vi "GOOP_ClassTool.vi"(0 "ClassRef":refnum<vi>, 5 "Error In":errorcluster) -> (19 "Error Out":errorcluster)   [LabVIEW 2020]
uses:
  ClassProviders/Common/ScriptingFunctions/Scripting_ConnectorPanePatternType.ctl
  <vilib>/Utility/miscctls.llb/LVPositionTypeDef.ctl
  API/GDSAPI_CreateInterfaceType.ctl
  ClassProviders/Provider_BaseClassInterface/ClassWriter_class/InterfaceMethodsToCreate.ctl
  ClassProviders/Common/CommonVIs/CommonVIs_AttributeType.ctl
  ClassProviders/Common/CommonVIs/CommonVIs_AttributeDataType.ctl
  ClassProviders/Common/String/GDSString_AccessScopeModifierType.ctl
  ClassProviders/Provider_EndevoGOOP300/GOOP300_SubVIs/GOOP300_MethodScopeType.ctl
  API/GDSAPI_SubVIs/GDSAPI_MethodType.ctl
  <vilib>/regexp/Match Regular Expression.xnode
  ClassProviders/Common/ScriptingFunctions/Scripting.lvclass
  ClassProviders/Provider_BaseClassInterface/ClassWriter_class/ClassWriter.lvclass
panel:
  in  "SelectAll":bool
  in  "ClassesCancel":bool
  in  "ClassesOK":bool
  in  "Classes":i32[](listbox)
  in  "MoreClasses":bool
  in  "Class(es)":u16(ring) items=["<Select Class(s)>", "-"]
  in  "Tab":enum32{"CP", "ClassControlName", "Interface"}(tab)
  in  "ApplyCP":bool
  in  "CP2":u16(ring) caption="To" items=["4x4x4", "5x6x5", "6x8x6"]
  out "CP1":T1 caption="From" items=["4x4x4", "5x6x5", "6x8x6"]
  out "ClassNameOut":string
  out "ClassNameIn":string
  in  "ClassControlName":string(combo) caption="New names of class controls and indicators"
  in  "UpdateClassControlNames":bool
  in  "InterfaceToCreate":u16(ring) caption="Select interface to create from current class..." items=["Create a parent class based on some of my methods of my class: AA", "Create an Interface(By VI Server) based on some of my methods of my class: AA", "Create an Interface and Adaptor class based on some of my methods of my class: AA"]
  out "InterfaceOptionTab":enum32{"Parent", "Adapter"}(tab)
  out "ReasonWhyParentClassCan'tBeCreated":string
  in  "CreateClassAndMethods":bool
  in  "ParentFolder":path
  in  "ParentClassName":string
  in  "ParentClass":u16(ring) items=["", "A", "AA-Base", "ABC", "B", "Base", "ClassWriter", "ClassWriterGOOP300", "ClassWriterGOOP400", "ClassWriterNative", "Scripting"]
  out "MyClassName(ParentClass)":string
  in  "MyClassMethods":i32[](listbox) caption="Class methods to add in the Parent class"
  out "Parent/InterafaceImage":u16(ring)
  in  "ParentMethodName":string
  out "MyClassName(InteraceClass)":string
  in  "AdaptorClassName":string
  in  "AdaptorFolder":path
  in  "Parent Methods":i32(listbox)
  in  "MyClassMethods(Interface)":i32[](listbox) caption="Class methods"
  in  "InterfaceClassName":string
  in  "InterfaceClass":u16(ring) items=["", "A", "B", "BBB", "CCC", "ClassWriter", "ClassWriterGOOP300", "ClassWriterGOOP400", "ClassWriterNative", "IA", "Scripting", "Top"]
  in  "InterfaceFolder":path
  out "ReasonWhyInterfaceClassCan'tBeCreated":string
  in  "CreateInterfaceAdaptorClassAndMethods":bool
  # "Select the Connector Pane you wish to change to and press CHANGE when done."
  # "Change the class reference control and indicator name. Press UPDATE when done."
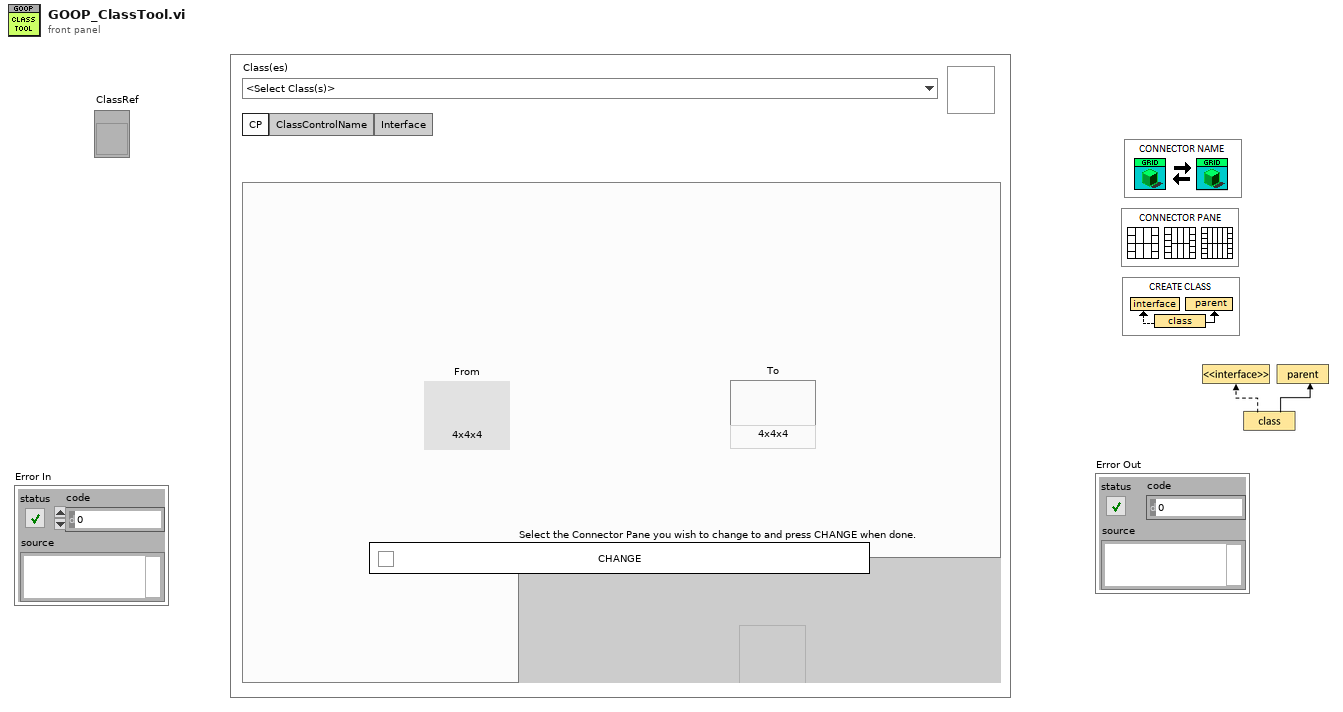
[diagram p1: front panel]
types:
  T1 = typedef "Scripting_ConnectorPanePatternType.ctl" = u16
  T2 = cluster{"Classes":refnum<vi>[], "Selected":i32[], "DropDownClasses":refnum<vi>[], "Interfaces":refnum<vi>[], "Methods":refnum<vi>[], "ExistingParentClassIdx":i32, "NewDropDownClassIdx":i32, "AdpUpdates":bool, "SelectClassPath":path, "ParentClassCreated":path, "NewClassCreated":bool}
  T3 = enum32{"Invalid", "Default", "Floating", "Floating/Auto-Hide", "Modal"}
  T4 = enum8{"Enabled", "Disabled", "Disabled and Grayed Out"}
  T5 = enum32{"invalid scope", "public", "private", "protected", "community"}
  T6 = typedef "LVPositionTypeDef.ctl" = cluster{"Left":i32, "Top":i32}
  T7 = typedef "GDSAPI_CreateInterfaceType.ctl" = cluster{"NewInterfaceFolder":path, "InterfaceName":string, "InterfaceDescription":string, "ParentInterfacesFilePath":path[], "FolderSuffix":string, "MethodsToCreate":T8[]}
  T8 = typedef "ClassWriter.lvclass/InterfaceMethodsToCreate.ctl" = cluster{"Name":string, "Description":string, "MethodsArgumentsIn":T9[], "MethodsArgumentsOut":T9[], "DecendantsMustOverride":bool}
  T9 = typedef "CommonVIs_AttributeType.ctl" = cluster{"Name":string, "DataType":T10, "ArrayDim":i32, "CtrlPath":path, "DataTypeString":string, "AccessScope":T11, "InitialData":variant}
  T10 = typedef "CommonVIs_AttributeDataType.ctl" = enum16{"UINT8", "INT8", "UINT16", "INT16", "UINT32", "INT32", "UINT64", "INT64", "SGL", "DBL", "EXT", "CSG", "CDB", "CXT", "TimeStamp", "STRING", "PATH", "BOOL", "ENUM", "RefNum", "VIRefNum", "LabVIEW Class", "Cluster", "Variant", "TypeDef", "Waveform", "LabVIEW Object", "Other", "void", "Set", "Map"}
  T11 = typedef "GDSString_AccessScopeModifierType.ctl" = enum16{"public", "private", "protected", "internal"}
  T12 = typedef "GOOP300_MethodScopeType.ctl" = enum16{"Use Parent Folder Scope", "Public", "Protected", "Private", "Community"}
  T13 = typedef "GDSAPI_MethodType.ctl" = enum16{"Read Attribute", "Write Attribute", "Read & Write Attribute", "None Modifying Method", "Get Property", "Set Property", "Read Property", "Write Property", "Static Method", "Interface Method"}
  T14 = cluster{"MethodName":string, "RelativeMethodPath":path, "MethodDescription":string, "Scope/Visibility":T12, "MethodType":T13, "RelativeProjectClassPath":string, "DynamicDispatchVi":bool, "OverrideMethod(Path)/PropertyMethod(AttributeName)":string}
  T15 = typedef "GDSLvCLass_ClassSettingsType.ctl" = cluster{"ClassProviderName":string, "ClassTemplateUsed":string, "ClassTemplateVersion":string, "ClassDescription":string, "PlugIns":T16[], "ConnectorPanePattern":string}
  T16 = typedef "GDSLvClass_PlugIn.ctl" = cluster{"Type":T17, "ID":string, "Version":string, "Path":path, "Name":string, "Data":variant}
  T17 = typedef "GDSLvClass_PlugInTypes.ctl" = enum16{"DesignPattern", "MethodTypes"}
  T18 = cluster{"result string":string, "ClassRef":refnum<vi>}
  T19 = cluster{"result string":string, "ClassRef":refnum<vi>}[]
  T20 = typedef "lveventtype.ctl" = enum32{"Null", "Timeout", "Annotation Menu Selection", "Annotation Menu Selection?", "App Instance Close", "App Instance Close?", "Autoscale Range Change", "Bookmark Info Change", "Cell Edit", "Cell Edit?", "Cursor Grab", "Cursor Grab?", "Cursor Menu Selection", "Cursor Menu Selection?", "Cursor Move", "Cursor Release", "Data Change", "Direction Change", "Display State Change", "Drag Ended", "Drag Enter", "Drag Leave", "Drag Over", "Drag Source Update", "Drag Starting", "Drag Starting?", "Drop", "Exec State Change", "Key Down", "Key Down?", "Key Repeat", "Key Repeat?", "Key Up", "Listbox Double Click", "Menu Activation?", "Menu Selection (App)", "Menu Selection? (App)", "Menu Selection (User)", "Mouse Down", "Mouse Down?", "Mouse Enter", "Mouse Leave", "Mouse Move", "Mouse Up", "Mouse Wheel", "NI Security User Change (App)", "Pane Size", "Panel Close", "Panel Close?", "Panel Resize", "Plot Attribute Change", "Scale Range Change", "Shortcut Menu Activation?", "Shortcut Menu Selection (App)", "Shortcut Menu Selection? (App)", "Shortcut Menu Selection (User)", "Tree Double Click", "Tree Drag", "Tree Drag?", "Tree Drop", "Tree Drop?", "Tree Item Close", "Tree Item Close?", "Tree Item Open", "Tree Item Open?", "User Event", "Value Change"}
  T21 = typedef "LVRowAndColumnUnsignedTypeDef.ctl" = cluster{"Row":u32, "Column":u32}
  T22 = cluster{"MethodName":string, "RelativeMethodPath":path, "MethodDescription":string, "Scope/Visibility":T12, "MethodType":T13, "RelativeProjectClassPath":string, "DynamicDispatchVi":bool, "OverrideMethod(Path)/PropertyMethod(AttributeName)":string}[]
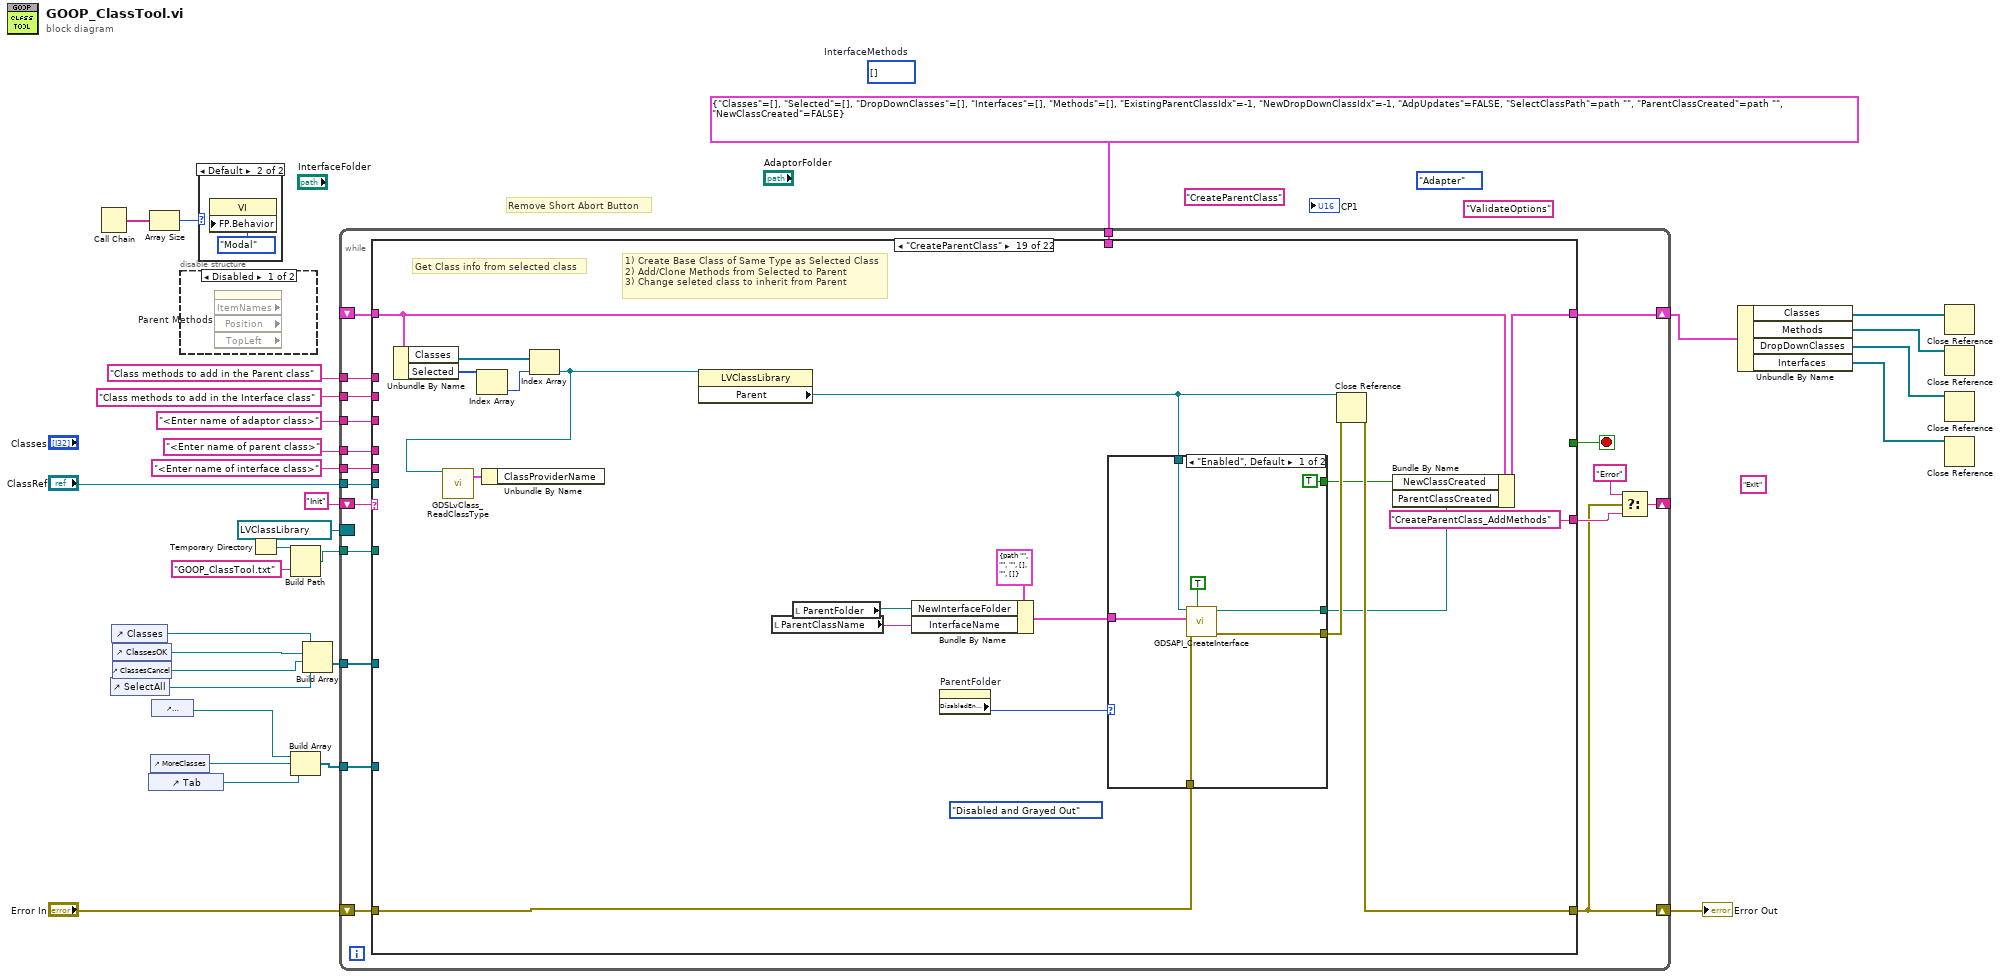
[diagram p0: block diagram]
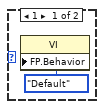
[diagram p3: hidden frame]
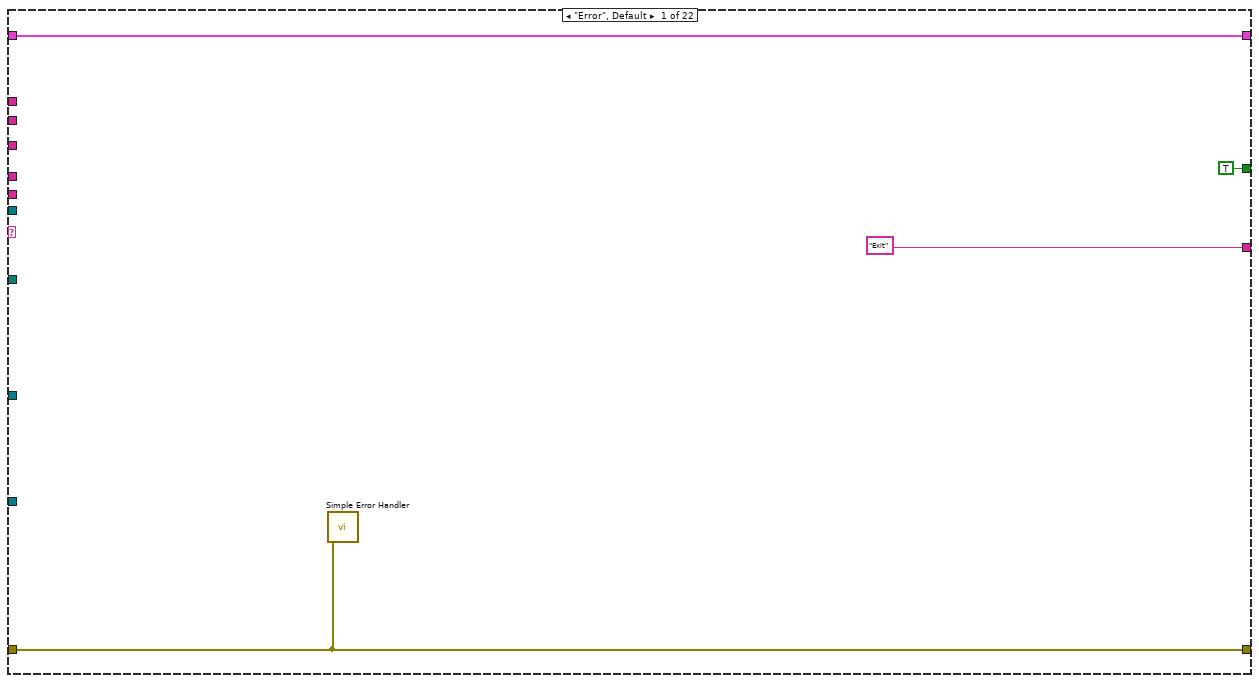
[diagram p4: hidden frame]
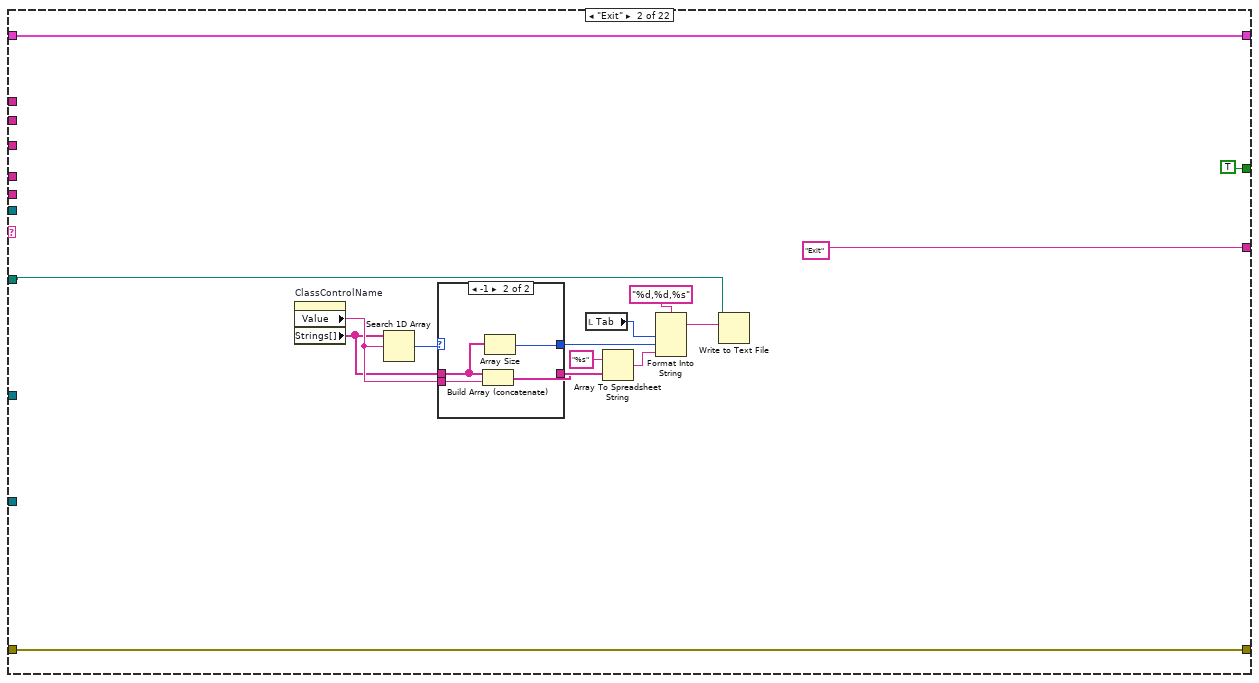
[diagram p5: hidden frame]
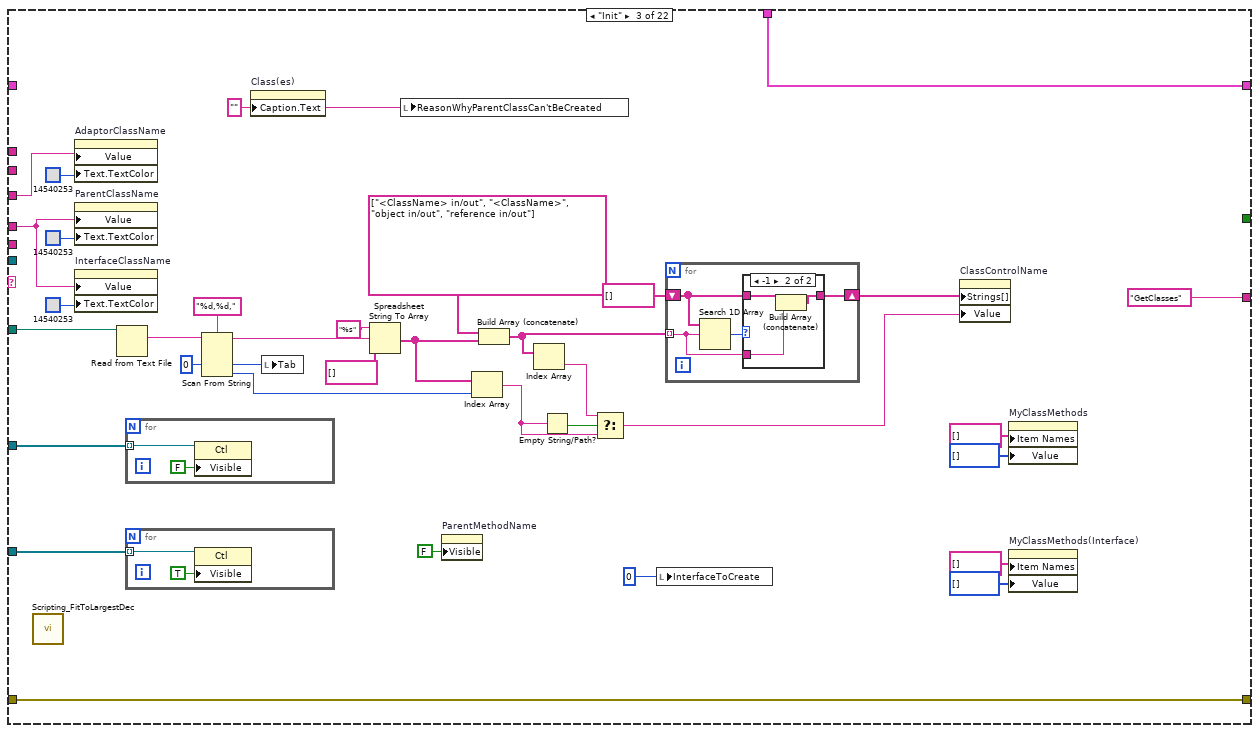
[diagram p7: hidden frame]
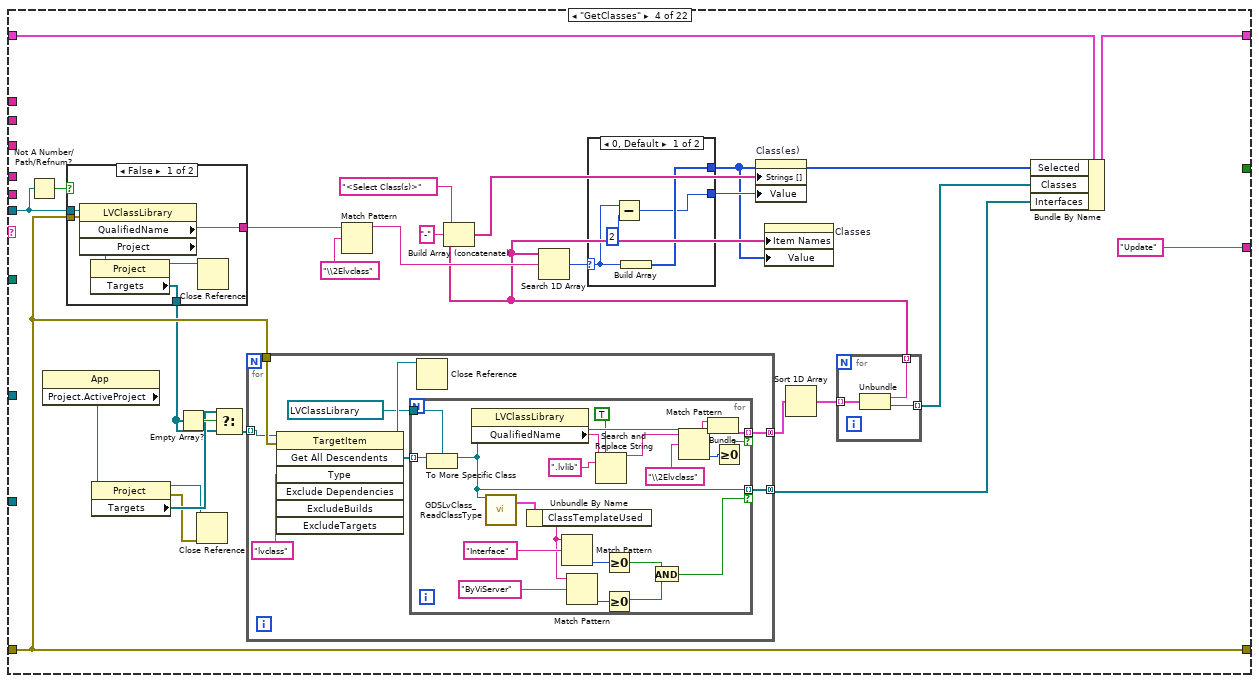
[diagram p9: hidden frame]
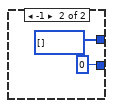
[diagram p10: hidden frame]
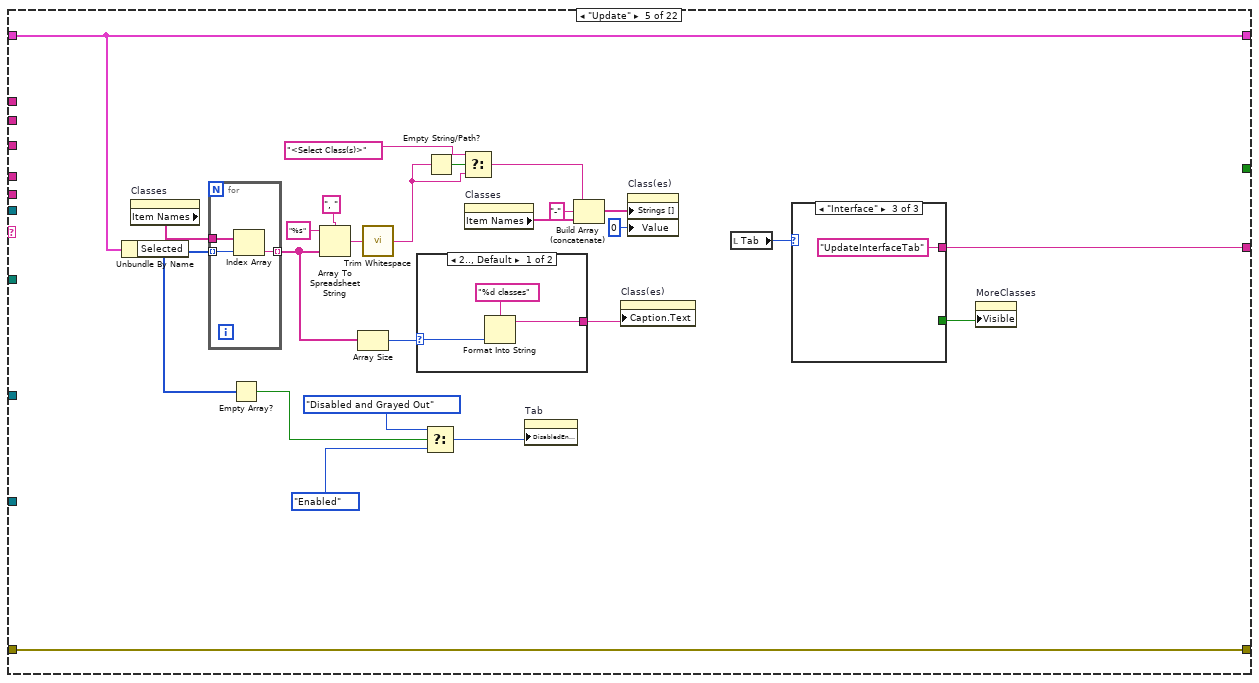
[diagram p12: hidden frame]
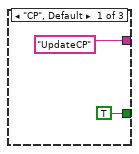
[diagram p13: hidden frame]
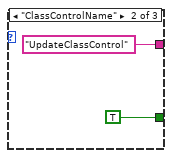
[diagram p14: hidden frame]
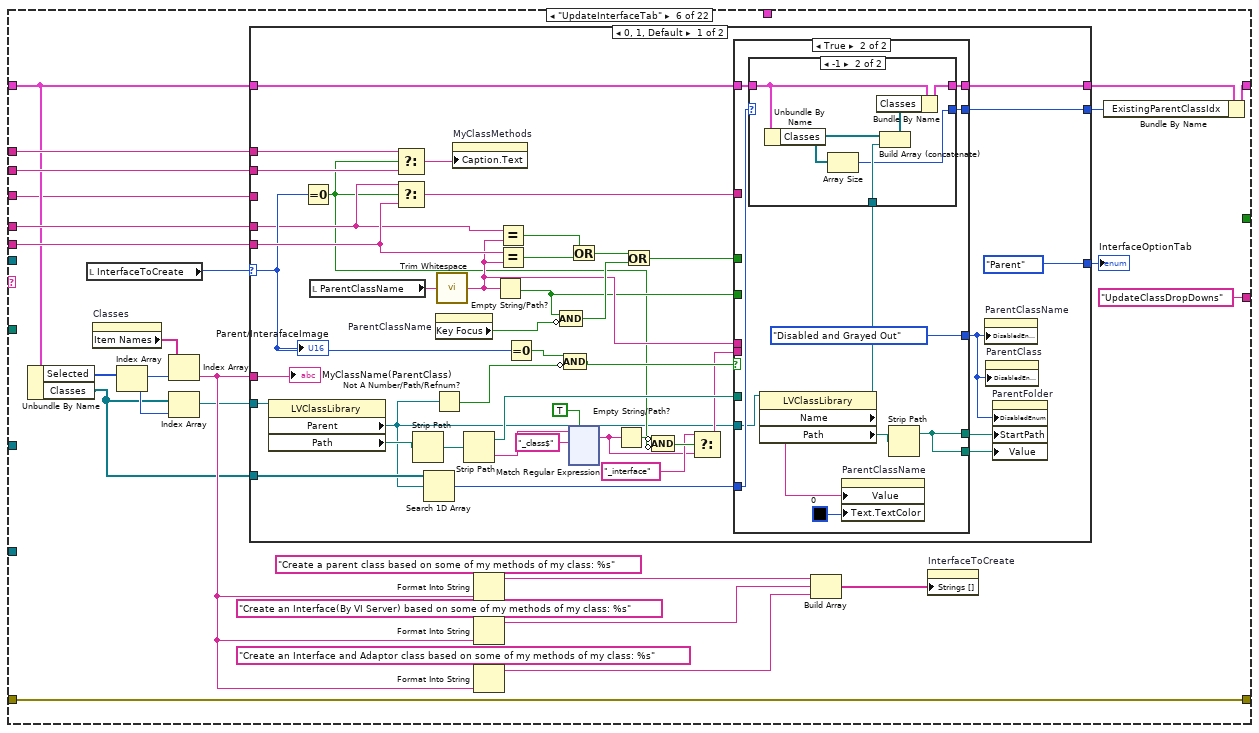
[diagram p16: hidden frame]
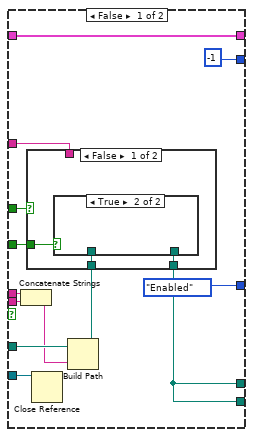
[diagram p17: hidden frame]
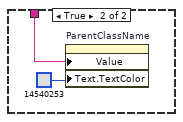
[diagram p19: hidden frame]
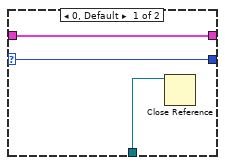
[diagram p20: hidden frame]
diagram:
  (unwired) "Exit"
  (unwired) "CreateParentClass"
  (unwired) "ValidateOptions"
  (unwired) enum32{"Parent", "Adapter"}."Adapter" ("InterfaceOptionTab")
  (unwired) i32[] []  # InterfaceMethods
  # "Remove Short Abort Button"
  n1 = Call Chain() -> (call chain=w7:string[])
  n2 = control-ref of="SelectAll"() -> (w18:refnum<vi>)
  n3 = control-ref of="Classes"() -> (w27:refnum<vi>)
  n4 = control-ref of="ClassesOK"() -> (w26:refnum<vi>)
  n5 = control-ref of="ClassesCancel"() -> (w25:refnum<vi>)
  n6 = control-ref of="Tab"() -> (w22:refnum<vi>)
  n7 = Array Size(array=w7) -> (size(s)=w6:i32)
  n8 = control-ref of="MoreClasses"() -> (w23:refnum<vi>)
  n9 = control-ref of="Class(es)"() -> (w17:refnum<vi>)
  n10 = disable-structure shown="Disabled" {
    frame Disabled {
      n11 = property on="Parent Methods" class="MCListbox (strict)" props=["ItemNames", "Position", "TopLeft"]() -> ()  [unwired: 2 in, 5 out]
    }
    frame Enabled {
    }
  }
  n12 = case shown="Default" w6 {
    frame 1 {
      n13 = property class="VI"("FP.Behavior"=T3."Default" ("Front Panel Window:Behavior")) -> ()  [unwired: 2 in, 2 out]
    }
    frame Default {
      n14 = property class="VI"("FP.Behavior"=T3."Modal" ("Front Panel Window:Behavior")) -> ()  [unwired: 2 in, 2 out]
    }
  }
  n15 = Temporary Directory() -> (w14:path)
  n16 = Build Path(base path=w14, name or relative path="GOOP_ClassTool.txt") -> (appended path=w13:path)
  n17 = Build Array(w17, w23, w22) -> (w21:refnum<vi>[])
  n18 = Build Array(w27, w26, w25, w18) -> (w24:refnum<vi>[])
  n19 = while {
    shift-right: [w46] -> w28
    shift-left: "Error In" -> [w51]
    shift-right: [w49] -> _
    shift-left: "Init" -> [w50]
    shift-right: [w45] -> w1
    shift-left: _ -> [w44]
    tunnel: w24 -> [w43]
    tunnel: w21 -> [w42]
    tunnel: "ClassRef" -> [w41]
    tunnel: T2 {"Classes"=[], "Selected"=[], "DropDownClasses"=[], "Interfaces"=[], "Methods"=[], "ExistingParentClassIdx"=-1, "NewDropDownClassIdx"=-1, "AdpUpdates"=FALSE, "SelectClassPath"=path "", "ParentClassCreated"=path "", "NewClassCreated"=FALSE} -> [w40]
    tunnel: w13 -> [w39]
    tunnel: "<Enter name of parent class>" ("ParentClassName") -> [w37]
    tunnel: "<Enter name of interface class>" ("ParentClassName") -> [w36]
    tunnel: "Class methods to add in the Parent class" ("Caption.Text") -> [w35]
    tunnel: "Class methods to add in the Interface class" ("Caption.Text") -> [w34]
    border: refnum<vi> refnum ("ClassRef") -> [_]
    tunnel: "<Enter name of adaptor class>" ("ParentClassName") -> [w33]
    stop <- w38 stop-if-true
    n20 = case shown="\"CreateParentClass\"" w50 {
      tunnel: w51 -> [w52 w70 w110 w133 w220 w247 w641 w722 w772 w799 w939 w1053 w1102 w1477 w1486 w1504 w1546 w1671 w1678 w1712 w1740 w1749]
      tunnel: [w52 w70 w110 w133 w220 w247 w641 w722 w772 w799 w939 w1053 w1102 w1477 w1483 w1500 w1546 w1671 w1685 w1706 w1733 w1749] -> w46
      tunnel: ["Exit" "Exit" "GetClasses" "Update" w208 "UpdateClassDropDowns" "UpdateMethods" w710 "AutoUpdateAdaptorName" "ValidateOptions" _ _ w1103 "Update" "Done" "Done" _ _ "CreateParentClass_AddMethods" w1709 "Done" ("message") "Exit"] -> w47
      tunnel: [w54 w68 w107 w136 w209 w236 w640 w718 w773 w798 w937 w1052 w1104 w1478 w1487 w1507 w1545 w1672 w1684 w1708 w1731 w1747] -> w45
      tunnel: w44 -> [w54 w68 _ w149 w209 w235 w638 w719 w773 w798 w937 w1052 w1099 w1480 w1487 w1507 w1545 w1672 w1690 w1708 w1731 w1747]
      tunnel: w43 -> [_ _ w109 _ _ _ _ _ _ _ _ _ w1101 _ _ _ _ _ _ _ _ _]
      tunnel: w42 -> [_ _ w108 _ _ _ _ _ _ _ _ _ w1100 _ _ _ _ _ _ _ _ _]
      tunnel: w41 -> [_ _ _ w132 _ _ _ _ _ _ _ _ _ _ _ _ _ _ _ _ _ _]
      tunnel: w40 -> [_ _ w107 _ _ _ _ _ _ _ _ _ _ _ _ _ _ _ _ _ _ _]
      tunnel: w39 -> [_ w57 w99 _ _ _ _ _ _ _ _ _ _ _ _ _ _ _ _ _ _ _]
      tunnel: [TRUE TRUE _ _ _ _ _ _ _ _ _ _ _ _ _ _ _ _ _ _ _ _] -> w38
      tunnel: w37 -> [_ _ w81 _ _ w246 _ _ _ w796 w936 _ w1098 _ _ _ _ _ _ _ _ _]
      tunnel: w36 -> [_ _ _ _ _ w243 _ _ _ _ w935 _ w1096 _ _ _ _ _ _ _ _ _]
      tunnel: w35 -> [_ _ _ _ _ w239 _ _ _ _ _ _ _ _ _ _ _ _ _ _ _ _]
      tunnel: w34 -> [_ _ _ _ _ w238 _ _ _ _ _ _ _ _ _ _ _ _ _ _ _ _]
      tunnel: w33 -> [_ _ w78 _ _ w232 _ _ _ w795 _ _ w1095 _ _ _ _ _ _ _ _ _]
      frame "Error", Default {
        n21 = call <vilib>:"Simple Error Handler.vi"("error in (no error)"=w52) -> ()  [unwired: 4 in, 5 out]
      }
      frame "Exit" {
        n22 = property on="ClassControlName" class="CmbBox"() -> ("Value"=w62:string, "Strings[]"=w61:string[])  [unwired: 2 in, 2 out]
        n23 = Search 1D Array(1D array=w61, element=w62) -> (index of element=w58:i32)  [unwired: 1 in]
        n24 = case shown="-1" w58 {
          selector: w58 -> [w72 _]
          tunnel: [w72 w74] -> w59
          tunnel: w61 -> [w71 w75]
          tunnel: w62 -> [_ w76]
          tunnel: [w71 w73] -> w65
          frame 0, Default {
          }
          frame -1 {
            n25 = Build Array (concatenate)(w75, w76) -> (w73:string[])
            n26 = Array Size(array=w75) -> (size(s)=w74:i32)
          }
        }
        n27 = local read "Tab"() -> (w67:enum32{"CP", "ClassControlName", "Interface"})
        n28 = Array To Spreadsheet String(array=w65, 3:"%s" ("format string")) -> (spreadsheet string=w64:string)  [unwired: 1 in]
        n29 = Format Into String(format string="%d,%d,%s", w67, w59, w64) -> (resulting string=w66:string)  [unwired: 2 in, 1 out]
        n30 = Write to Text File(file (use dialog)=w57, text=w66) -> ()  [unwired: 2 in, 3 out]
      }
      frame "Init" {
        w80 = "" ("Caption.Text")
        n31 = call "Scripting_FitToLargestDec.vi"() -> ()  [unwired: 6 in, 2 out]
        n32 = property on="AdaptorClassName" class="Str"("Value"=w78, "Text.TextColor"=u32 14540253) -> ()  [unwired: 2 in, 2 out]
        n33 = property on="ParentClassName" class="Str"("Value"=w81, "Text.TextColor"=u32 14540253) -> ()  [unwired: 2 in, 2 out]
        n34 = property on="InterfaceClassName" class="Str"("Value"=w81, "Text.TextColor"=u32 14540253) -> ()  [unwired: 2 in, 2 out]
        n35 = Read from Text File(file (use dialog)=w99) -> (text=w106:string)  [unwired: 3 in, 3 out]
        n36 = for {
          tunnel: w109 -> [w123] mode=indexing
          n37 = property on="Property Node" class="Ctl"(reference=w123, "Visible"=FALSE) -> ()  [unwired: 1 in, 2 out]
        }
        n38 = for {
          tunnel: w108 -> [w121] mode=indexing
          n39 = property on="Property Node" class="Ctl"(reference=w121, "Visible"=TRUE) -> ()  [unwired: 1 in, 2 out]
        }
        n40 = Scan From String(format string="%d,%d,", input string=w106, default 1=0 ("default value 1")) -> (remaining string=w104:string, output 1=w97:i32, output 2=w95:i32)  [unwired: 3 in, 2 out]
        n41 = property on="Class(es)" class="Ring (strict)"("Caption.Text"=w80) -> ()  [unwired: 2 in, 2 out]
        n42 = local write "Tab"(w97) -> ()
        n43 = Spreadsheet String To Array(format string="%s", spreadsheet string=w104, array type (2D Dbl)=string[] []) -> (array=w96:string[])  [unwired: 1 in]
        n44 = local write "ReasonWhyParentClassCan'tBeCreated"(w80) -> ()
        n45 = property on="ParentMethodName" class="Str"("Visible"=FALSE) -> ()  [unwired: 2 in, 2 out]
        n46 = Index Array(array=w96, index=w95) -> (element=w90:string)
        n47 = Build Array (concatenate)(string[] ["<ClassName> in/out", "<ClassName>", "object in/out", "reference in/out"] ("Strings []"), w96) -> (w93:string[])
        n48 = Index Array(array=w93) -> (element=w91:string)  [unwired: 1 in]
        n49 = Empty String/Path?(string/path=w90) -> (empty?=w92:bool)
        n50 = Select(t=w91, s=w92, f=w90) -> (s? t:f=w89:string)
        n51 = local write "InterfaceToCreate"(0) -> ()
        n52 = for {
          tunnel: w93 -> [w113] mode=indexing
          shift-right: [w112] -> w94
          shift-left: string[] [] -> [w114]
          n53 = Search 1D Array(1D array=w114, element=w113) -> (index of element=w115:i32)  [unwired: 1 in]
          n54 = case shown="-1" w115 {
            tunnel: w114 -> [w116 w119]
            tunnel: w113 -> [_ w118]
            tunnel: [w116 w117] -> w112
            frame 0, Default {
            }
            frame -1 {
              n55 = Build Array (concatenate)(w119, w118) -> (w117:string[])
            }
          }
        }
        n56 = property on="ClassControlName" class="CmbBox"("Strings[]"=w94, "Value"=w89) -> ()  [unwired: 2 in, 2 out]
        n57 = property on="MyClassMethods" class="LstBox (strict)"("Item Names"=string[] [], "Value"=i32[] [] ("MyClassMethods")) -> ()  [unwired: 2 in, 2 out]
        n58 = property on="MyClassMethods(Interface)" class="LstBox (strict)"("Item Names"=string[] [], "Value"=i32[] [] ("MyClassMethods")) -> ()  [unwired: 2 in, 2 out]
      }
      frame "GetClasses" {
        n59 = Not A Number/Path/Refnum?(number/path/refnum=w132) -> (NaN/Path/Refnum?=w131:bool)
        n60 = property class="App"() -> ("Project.ActiveProject"=w130:refnum<vi>)  [unwired: 2 in, 2 out]
        n61 = case shown="False" w131 {
          tunnel: [w162 _] -> w148
          tunnel: [w160 _] -> w129
          tunnel: w133 -> [w159 _]
          tunnel: w132 -> [w158 _]
          frame False {
            n62 = property class="LVClassLibrary"(reference=w158, error in=w159) -> ("QualifiedName"=w162:string, "Project"=w161:refnum<vi>)  [unwired: 2 out]
            n63 = property class="Project"(reference=w161) -> (reference out=w157:refnum<vi>, "Targets"=w160:refnum<vi>[])  [unwired: 1 in, 1 out]
            n64 = Close Reference(reference=w157) -> ()  [unwired: 1 in, 1 out]
          }
          frame True {
          }
        }
        n65 = property class="Project"(reference=w130) -> (reference out=w125:refnum<vi>, error out=w126:errorcluster, "Targets"=w141:refnum<vi>[])  [unwired: 1 in]
        n66 = Empty Array?(array=w129) -> (empty?=w142:bool)
        n67 = Close Reference(reference=w125, error in (no error)=w126) -> ()  [unwired: 1 out]
        n68 = Select(t=w141, s=w142, f=w129) -> (s? t:f=w140:refnum<vi>[])
        n69 = for {
          tunnel: [w171] -> w144 mode=concatenating
          tunnel: w133 -> [w170]
          tunnel: w140 -> [w169] mode=indexing
          tunnel: [w166] -> w124 mode=concatenating
          n70 = invoke class="TargetItem" method="Get All Descendents"(reference=w169, error in=w170, "Type"="lvclass") -> (reference out=w168:refnum<vi>, "All Descendents"=w172:refnum<vi>[])  [unwired: 4 in, 5 out]
          n71 = for {
            tunnel: w172 -> [w195] mode=indexing
            tunnel: [w189] -> w171 mode=indexing if=w192
            tunnel: refnum<vi> refnum ("ClassRef") -> [w184]
            tunnel: [w175] -> w166 mode=indexing if=w174
            n72 = To More Specific Class(target class=w184, reference=w195) -> (specific class reference=w175:refnum<vi>)  [unwired: 1 in, 1 out]
            n73 = property class="LVClassLibrary"(reference=w175) -> (reference out=w190:refnum<vi>, "QualifiedName"=w188:string)  [unwired: 1 in, 1 out]
            n74 = call "GDSLvClass_ReadClassType.vi"("Class Refnum In"=w175) -> ("ClassSettings"=w181:T15)  [unwired: 16 in, 2 out]
            n75 = Unbundle By Name(w181) -> ("ClassTemplateUsed"=w178:string)
            n76 = Match Pattern(string=w178, regular expression="Interface") -> (offset past match=w179:i32)  [unwired: 1 in, 3 out]
            n77 = Match Pattern(string=w178, regular expression="ByViServer") -> (offset past match=w176:i32)  [unwired: 1 in, 3 out]
            n78 = Search and Replace String(replace all?=TRUE ("replace all? (F)"), input string=w188, search string=".lvlib" ("regular expression")) -> (result string=w187:string)  [unwired: 5 in, 3 out]
            n79 = Greater Or Equal To 0?(x=w179) -> (x >= 0?=w182:bool)
            n80 = Greater Or Equal To 0?(x=w176) -> (x >= 0?=w183:bool)
            n81 = And(x=w182, y=w183) -> (x .and. y?=w174:bool)
            n82 = Match Pattern(string=w187, regular expression="\\2Elvclass") -> (before substring=w191:string, offset past match=w193:i32)  [unwired: 1 in, 2 out]
            n83 = Bundle("result string"=w191, "ClassRef"=w190) -> (w189:T18)  [unwired: 1 in]
            n84 = Greater Or Equal To 0?(x=w193) -> (x >= 0?=w192:bool)
          }
          n85 = Close Reference(reference=w168) -> ()  [unwired: 1 in, 1 out]
        }
        n86 = Match Pattern(string=w148, regular expression="\\2Elvclass") -> (before substring=w139:string)  [unwired: 1 in, 3 out]
        n87 = Sort 1D Array(array=w144) -> (sorted array=w138:T19)
        n88 = for {
          tunnel: w138 -> [w165] mode=indexing
          tunnel: [w164] -> w135 mode=indexing
          tunnel: [w163] -> w137 mode=indexing
          n89 = Unbundle(w165) -> ("result string"=w163:string, "ClassRef"=w164:refnum<vi>)
        }
        n90 = Build Array (concatenate)("<Select Class(s)>" ("element"), "-" ("element"), w137) -> (w145:string[])
        n91 = Search 1D Array(1D array=w137, element=w139) -> (index of element=w128:i32)  [unwired: 1 in]
        n92 = case shown="0, Default" w128 {
          selector: w128 -> [w154 _]
          tunnel: [w151 0 ("Classes")] -> w143
          tunnel: [w153 i32[] [] ("Classes")] -> w127
          frame 0, Default {
            n93 = Subtract(x=w154, y=2) -> (x-y=w151:i32)
            n94 = Build Array(w154) -> (w153:i32[])
          }
          frame -1 {
          }
        }
        n95 = property on="Class(es)" class="Ring (strict)"("Strings []"=w145, "Value"=w143) -> ()  [unwired: 2 in, 2 out]
        n96 = property on="Classes" class="LstBox (strict)"("Item Names"=w137, "Value"=w127) -> ()  [unwired: 2 in, 2 out]
        n97 = Bundle By Name(cluster=w149, "Selected"=w127, "Classes"=w135, "Interfaces"=w124) -> (w136:T2)
      }
      frame "Update" {
        n98 = Unbundle By Name(w209) -> ("Selected"=w207:i32[])
        n99 = property on="Classes" class="LstBox (strict)"() -> ("Item Names"=w219:string[])  [unwired: 2 in, 2 out]
        n100 = for {
          tunnel: w207 -> [w231] mode=indexing
          tunnel: w219 -> [w230]
          tunnel: [w229] -> w196 mode=indexing
          n101 = Index Array(array=w230, index=w231) -> (element=w229:string)
        }
        n102 = Empty Array?(array=w207) -> (empty?=w206:bool)
        n103 = Array To Spreadsheet String(delimiter (Tab)=", ", array=w196, 3:"%s" ("format string")) -> (spreadsheet string=w216:string)
        n104 = Array Size(array=w196) -> (size(s)=w215:i32)
        n105 = call <vilib>:"Trim Whitespace.vi"("string"=w216) -> ("trimmed string"=w200:string)  [unwired: 1 in]
        n106 = case shown="2.., Default" w215 {
          selector: w215 -> [w228 _]
          tunnel: [w226 _] -> w214
          frame 2.., Default {
            n107 = Format Into String(format string="%d classes", w228) -> (resulting string=w226:string)  [unwired: 2 in, 1 out]
          }
          frame ..1 {
          }
        }
        n108 = Select(t=T4."Disabled and Grayed Out", s=w206, f=T4."Enabled" ("Disabled")) -> (s? t:f=w203:T4)
        n109 = Empty String/Path?(string/path=w200) -> (empty?=w202:bool)
        n110 = Select(t="<Select Class(s)>" ("element"), s=w202, f=w200) -> (s? t:f=w199:string)
        n111 = property on="Classes" class="LstBox (strict)"() -> ("Item Names"=w213:string[])  [unwired: 2 in, 2 out]
        n112 = property on="Tab" class="TabCtl (strict)"("DisabledEnum"=w203) -> ()  [unwired: 2 in, 2 out]
        n113 = Build Array (concatenate)(w199, "-" ("element"), w213) -> (w212:string[])
        n114 = property on="Class(es)" class="Ring (strict)"("Caption.Text"=w214) -> ()  [unwired: 2 in, 2 out]
        n115 = property on="Class(es)" class="Ring (strict)"("Strings []"=w212, "Value"=0 ("Classes")) -> ()  [unwired: 2 in, 2 out]
        n116 = local read "Tab"() -> (w198:enum32{"CP", "ClassControlName", "Interface"})
        n117 = case shown="\"Interface\"" w198 {
          tunnel: ["UpdateCP" "UpdateClassControl" "UpdateInterfaceTab"] -> w208
          tunnel: [TRUE TRUE _] -> w197
          frame "CP", Default {
          }
          frame "ClassControlName" {
          }
          frame "Interface" {
          }
        }
        n118 = property on="MoreClasses" class="Bool"("Visible"=w197) -> ()  [unwired: 2 in, 2 out]
      }
      frame "UpdateInterfaceTab" {
        n119 = Unbundle By Name(w235) -> ("Selected"=w257:i32[], "Classes"=w237:refnum<vi>[])
        n120 = local read "InterfaceToCreate"() -> (w244:u16)
        n121 = property on="Classes" class="LstBox (strict)"() -> ("Item Names"=w256:string[])  [unwired: 2 in, 2 out]
        n122 = Index Array(array=w257) -> (element=w241:i32)  [unwired: 1 in]
        n123 = Index Array(array=w256, index=w241) -> (element=w248:string)
        n124 = Index Array(array=w237, index=w241) -> (element=w240:refnum<vi>)
        n125 = case shown="0, 1, Default" w244 {
          selector: w244 -> [w287 w485]
          tunnel: w248 -> [w300 w470]
          tunnel: w246 -> [w275 w469]
          tunnel: [enum32{"Parent", "Adapter"}."Parent" ("InterfaceOptionTab") enum32{"Parent", "Adapter"}."Adapter" ("InterfaceOptionTab")] -> w245
          tunnel: w243 -> [w292 _]
          tunnel: w240 -> [w290 w489]
          tunnel: w239 -> [w274 _]
          tunnel: w238 -> [w273 _]
          tunnel: w237 -> [w263 _]
          tunnel: w235 -> [w260 w468]
          tunnel: [w259 w468] -> w234
          tunnel: [w258 -1 ("index of element")] -> w233
          tunnel: w232 -> [_ w456]
          frame 0, 1, Default {
            n126 = property class="LVClassLibrary"(reference=w290) -> ("Parent"=w262:refnum<vi>, "Path"=w284:path)  [unwired: 1 in, 2 out]
            n127 = Equal To 0?(x=w287) -> (x = 0?=w269:bool)
            n128 = local read "ParentClassName"() -> (w299:string)
            n129 = Select(t=w274, s=w269, f=w273) -> (s? t:f=w272:string)
            n130 = Select(t=w275, s=w269, f=w292) -> (s? t:f=w291:string)
            n131 = Strip Path(path=w284) -> (stripped path=w283:path)  [unwired: 1 out]
            n132 = Search 1D Array(1D array=w263, element=w262) -> (index of element=w261:i32)  [unwired: 1 in]
            n133 = Not A Number/Path/Refnum?(number/path/refnum=w262) -> (NaN/Path/Refnum?=w288:bool)
            n134 = property on="ParentClassName" class="Str"() -> ("Key Focus"=w298:bool)  [unwired: 2 in, 2 out]
            n135 = call <vilib>:"Trim Whitespace.vi"("string"=w299) -> ("trimmed string"=w277:string)  [unwired: 1 in]
            n136 = property on="MyClassMethods" class="LstBox (strict)"("Caption.Text"=w272) -> ()  [unwired: 2 in, 2 out]
            n137 = Strip Path(path=w283) -> (stripped path=w276:path, name=w280:string)
            n138 = Empty String/Path?(string/path=w277) -> (empty?=w271:bool)
            n139 = Equal?(x=w275, y=w277) -> (x = y?=w294:bool)
            n140 = Equal?(x=w292, y=w277) -> (x = y?=w295:bool)
            n141 = Equal To 0?(x=w287) -> (x = 0?=w286:bool)
            n142 = Compound Arithmetic op=AND(w271, invert w298) -> (w297:bool)
            n143 = Compound Arithmetic op=AND(w286, invert w288) -> (w285:bool)
            n144 = Or(x=w294, y=w295) -> (x .or. y?=w293:bool)
            n145 = xnode "Match Regular Expression"("input string"=w280, "regular expression"="_class$", "ignore case? (F)"=TRUE) -> ("whole match"=w266:string)  [unwired: 3 in, 4 out]
            n146 = Empty String/Path?(string/path=w266) -> (empty?=w270:bool)
            n147 = Or(x=w293, y=w297) -> (x .or. y?=w289:bool)
            n148 = Compound Arithmetic op=AND(invert w270, invert w269) -> (w268:bool)
            n149 = Select(t="_interface" ("regular expression"), s=w268, f=w266) -> (s? t:f=w265:string)
            n150 = case shown="True" w285 {
              tunnel: w291 -> [w427 _]
              tunnel: w262 -> [w425 w436]
              tunnel: w289 -> [w426 _]
              tunnel: [T4."Enabled" ("Disabled") T4."Disabled and Grayed Out" ("Disabled")] -> w264
              tunnel: [w419 w440] -> w282
              tunnel: [w419 w440] -> w281
              tunnel: w277 -> [w424 _]
              tunnel: w265 -> [w423 _]
              tunnel: w276 -> [w422 _]
              tunnel: w271 -> [w417 _]
              tunnel: w261 -> [_ w439]
              tunnel: w260 -> [w416 w438]
              tunnel: [w416 w437] -> w259
              tunnel: [-1 ("index of element") w435] -> w258
              frame False {
                n151 = Concatenate Strings(w424, w423) -> (w421:string)
                n152 = Close Reference(reference=w425) -> ()  [unwired: 1 in, 1 out]
                n153 = Build Path(base path=w422, name or relative path=w421) -> (appended path=w420:path)
                n154 = case shown="False" w426 {
                  tunnel: w427 -> [_ w432]
                  tunnel: w420 -> [w429 _]
                  tunnel: [w428 _] -> w419
                  tunnel: w417 -> [w430 _]
                  frame False {
                    n155 = case shown="True" w430 {
                      tunnel: w429 -> [w431 _]
                      tunnel: [w431 _] -> w428
                      frame False {
                      }
                      frame True {
                      }
                    }
                  }
                  frame True {
                    n156 = property on="ParentClassName" class="Str"("Value"=w432, "Text.TextColor"=u32 14540253) -> ()  [unwired: 2 in, 2 out]
                  }
                }
              }
              frame True {
                n157 = property class="LVClassLibrary"(reference=w436) -> (reference out=w434:refnum<vi>, "Name"=w442:string, "Path"=w441:path)  [unwired: 1 in, 1 out]
                n158 = case shown="-1" w439 {
                  selector: w439 -> [w445 _]
                  tunnel: w438 -> [w447 w452]
                  tunnel: [w447 w453] -> w437
                  tunnel: w434 -> [w446 w450]
                  tunnel: [w445 w448] -> w435
                  frame 0, Default {
                    n159 = Close Reference(reference=w446) -> ()  [unwired: 1 in, 1 out]
                  }
                  frame -1 {
                    n160 = Unbundle By Name(w452) -> ("Classes"=w449:refnum<vi>[])
                    n161 = Array Size(array=w449) -> (size(s)=w448:i32)
                    n162 = Build Array (concatenate)(w449, w450) -> (w451:refnum<vi>[])
                    n163 = Bundle By Name(cluster=w452, "Classes"=w451) -> (w453:T2)
                  }
                }
                n164 = property on="ParentClassName" class="Str"("Value"=w442, "Text.TextColor"=u32 0) -> ()  [unwired: 2 in, 2 out]
                n165 = Strip Path(path=w441) -> (stripped path=w440:path)  [unwired: 1 out]
              }
            }
            n166 = property on="ParentClassName" class="Str"("DisabledEnum"=w264) -> ()  [unwired: 2 in, 2 out]
            n167 = property on="ParentClass" class="Ring (strict)"("DisabledEnum"=w264) -> ()  [unwired: 2 in, 2 out]
            n168 = property on="ParentFolder" class="Path"("DisabledEnum"=w264, "StartPath"=w282, "Value"=w281) -> ()  [unwired: 2 in, 2 out]
            "MyClassName(ParentClass)" <- w300
            "Parent/InterafaceImage" <- w287
          }
          frame 2 {
            n169 = property class="LVClassLibrary"(reference=w489) -> ("Parent"=w488:refnum<vi>, "Path"=w482:path)  [unwired: 1 in, 2 out]
            n170 = local read "AdaptorClassName"() -> (w465:string)
            n171 = Equal To 0?(x=w485) -> (x = 0?=w472:bool)
            n172 = local read "InterfaceClassName"() -> (w492:string)
            n173 = property on="AdaptorClassName" class="Str"() -> ("Key Focus"=w462:bool)  [unwired: 2 in, 2 out]
            n174 = Strip Path(path=w482) -> (stripped path=w481:path)  [unwired: 1 out]
            n175 = call <vilib>:"Trim Whitespace.vi"("string"=w465) -> ("trimmed string"=w464:string)  [unwired: 1 in]
            n176 = Not A Number/Path/Refnum?(number/path/refnum=w488) -> (NaN/Path/Refnum?=w486:bool)
            n177 = property on="InterfaceClassName" class="Str"() -> ("Key Focus"=w491:bool)  [unwired: 2 in, 2 out]
            n178 = call <vilib>:"Trim Whitespace.vi"("string"=w492) -> ("trimmed string"=w475:string)  [unwired: 1 in]
            n179 = Strip Path(path=w481) -> (stripped path=w454:path, name=w478:string)
            n180 = Equal?(x=w464, y=w456) -> (x = y?=w463:bool)
            n181 = Empty String/Path?(string/path=w464) -> (empty?=w457:bool)
            n182 = Empty String/Path?(string/path=w475) -> (empty?=w474:bool)
            n183 = Equal?(x=w469, y=w475) -> (x = y?=w459:bool)
            n184 = Equal To 0?(x=w485) -> (x = 0?=w484:bool)
            n185 = Compound Arithmetic op=AND(invert w462, w457) -> (w461:bool)
            n186 = Or(x=w461, y=w463) -> (x .or. y?=w458:bool)
            n187 = Compound Arithmetic op=AND(w474, invert w491) -> (w460:bool)
            n188 = Compound Arithmetic op=AND(w484, invert w486) -> (w483:bool)
            n189 = xnode "Match Regular Expression"("input string"=w478, "regular expression"="_class$", "ignore case? (F)"=TRUE) -> ("whole match"=w466:string)  [unwired: 3 in, 4 out]
            n190 = Empty String/Path?(string/path=w466) -> (empty?=w473:bool)
            n191 = Compound Arithmetic op=AND(invert w473, invert w472) -> ()  [unwired: 1 out]
            n192 = Or(x=w459, y=w460) -> (x .or. y?=w487:bool)
            n193 = case shown="True" w483 {
              tunnel: w469 -> [w623 _]
              tunnel: w488 -> [w621 w635]
              tunnel: w487 -> [w622 _]
              tunnel: [T4."Enabled" ("Disabled") T4."Disabled and Grayed Out" ("Disabled")] -> w471
              tunnel: [w615 w630] -> w480
              tunnel: [w615 w630] -> w479
              tunnel: w475 -> [w620 _]
              tunnel: w466 -> [w619 _]
              tunnel: w454 -> [w618 _]
              tunnel: w474 -> [w613 _]
              frame False {
                n194 = Concatenate Strings(w620, w619) -> (w617:string)
                n195 = Close Reference(reference=w621) -> ()  [unwired: 1 in, 1 out]
                n196 = Build Path(base path=w618, name or relative path=w617) -> (appended path=w616:path)
                n197 = case shown="True" w622 {
                  tunnel: w623 -> [_ w628]
                  tunnel: w616 -> [w625 _]
                  tunnel: [w624 _] -> w615
                  tunnel: w613 -> [w626 _]
                  frame False {
                    n198 = case shown="False" w626 {
                      tunnel: w625 -> [w627 _]
                      tunnel: [w627 _] -> w624
                      frame False {
                      }
                      frame True {
                      }
                    }
                  }
                  frame True {
                    n199 = property on="InterfaceClassName" class="Str"("Value"=w628, "Text.TextColor"=u32 14540253) -> ()  [unwired: 2 in, 2 out]
                  }
                }
              }
              frame True {
                n200 = property class="LVClassLibrary"(reference=w635) -> (reference out=w636:refnum<vi>, "Name"=w632:string, "Path"=w631:path)  [unwired: 1 in, 1 out]
                n201 = property on="InterfaceClassName" class="Str"("Value"=w632, "Text.TextColor"=u32 0) -> ()  [unwired: 2 in, 2 out]
                n202 = Strip Path(path=w631) -> (stripped path=w630:path)  [unwired: 1 out]
                n203 = Close Reference(reference=w636) -> ()  [unwired: 1 in, 1 out]
              }
            }
            n204 = case shown="False" w458 {
              tunnel: w454 -> [w494 _]
              tunnel: [w493 _] -> w455
              tunnel: w457 -> [w495 _]
              tunnel: w456 -> [_ w497]
              frame False {
                n205 = case shown="True" w495 {
                  tunnel: w494 -> [w496 _]
                  tunnel: [w496 _] -> w493
                  frame False {
                  }
                  frame True {
                  }
                }
              }
              frame True {
                n206 = property on="AdaptorClassName" class="Str"("Value"=w497, "Text.TextColor"=u32 14540253) -> ()  [unwired: 2 in, 2 out]
              }
            }
            n207 = property on="InterfaceClassName" class="Str"("DisabledEnum"=w471) -> ()  [unwired: 2 in, 2 out]
            n208 = property on="InterfaceClass" class="Ring (strict)"("DisabledEnum"=w471) -> ()  [unwired: 2 in, 2 out]
            n209 = property on="AdaptorFolder" class="Path"("StartPath"=w455, "Value"=w455) -> ()  [unwired: 2 in, 2 out]
            n210 = property on="InterfaceFolder" class="Path"("DisabledEnum"=w471, "StartPath"=w480, "Value"=w479) -> ()  [unwired: 2 in, 2 out]
            "MyClassName(InteraceClass)" <- w470
          }
        }
        "InterfaceOptionTab" <- w245
        n211 = Format Into String(format string="Create a parent class based on some of my methods of my class: %s", w248) -> (resulting string=w254:string)  [unwired: 2 in, 1 out]
        n212 = Format Into String(format string="Create an Interface(By VI Server) based on some of my methods of my class: %s", w248) -> (resulting string=w251:string)  [unwired: 2 in, 1 out]
        n213 = Format Into String(format string="Create an Interface and Adaptor class based on some of my methods of my class: %s", w248) -> (resulting string=w249:string)  [unwired: 2 in, 1 out]
        n214 = Build Array(w254, w251, w249) -> (w253:string[])
        n215 = property on="InterfaceToCreate" class="Ring (strict)"("Strings []"=w253) -> ()  [unwired: 2 in, 2 out]
        n216 = Bundle By Name(cluster=w234, "ExistingParentClassIdx"=w233) -> (w236:T2)
      }
      frame "UpdateClassDropDowns" {
        n217 = local read "InterfaceToCreate"() -> (w642:u16)
        n218 = case shown="0, Default" w642 {
          tunnel: [w649 w687 w698] -> w639
          tunnel: w638 -> [w645 w691 w699]
          frame 0, Default {
            n219 = Unbundle By Name(w645) -> ("Classes"=w644:refnum<vi>[], "Selected"=w643:i32[])
            n220 = Index Array(array=w643) -> (element=w646:i32)  [unwired: 1 in]
            n221 = Index Array(array=w644, index=w646) -> (element=w651:refnum<vi>)
            n222 = property class="LVClassLibrary"(reference=w651) -> ("Name"=w653:string)  [unwired: 1 in, 2 out]
            n223 = for {
              tunnel: w644 -> [w667] mode=indexing
              tunnel: w653 -> [w662]
              shift-right: [w658] -> w649
              shift-left: refnum<vi>[] [] -> [w660]
              n224 = property class="LVClassLibrary"(reference=w667) -> (reference out=w659:refnum<vi>, "Name"=w665:string)  [unwired: 1 in, 1 out]
              n225 = Build Array(w665) -> (w664:string[])
              n226 = while {
                shift-right: [w674] -> w666
                shift-left: w659 -> [w680]
                shift-right: [w675] -> w663
                shift-left: w664 -> [w677]
                i -> [w672]
                stop <- w678 stop-if-true
                n227 = property class="LVClassLibrary"(reference=w680) -> (reference out=w673:refnum<vi>, error out=w679:errorcluster, "Parent"=w674:refnum<vi>)  [unwired: 1 in]
                n228 = case shown="1.." w672 {
                  tunnel: w673 -> [_ w681]
                  frame Default {
                  }
                  frame 1.. {
                    n229 = Close Reference(reference=w681) -> ()  [unwired: 1 in, 1 out]
                  }
                }
                n230 = property class="LVClassLibrary"(reference=w674, error in=w679) -> (error out=w678:errorcluster, "Name"=w676:string)  [unwired: 1 out]
                n231 = case shown="No Error" w678 {
                  tunnel: w677 -> [w684 w685]
                  tunnel: w676 -> [w683 _]
                  tunnel: [w682 w685] -> w675
                  frame No Error {
                    n232 = Build Array (concatenate)(w684, w683) -> (w682:string[])
                  }
                  frame Error {
                  }
                }
              }
              n233 = Close Reference(reference=w666) -> ()  [unwired: 1 in, 1 out]
              n234 = Search 1D Array(1D array=w663, element=w662) -> (index of element=w661:i32)  [unwired: 1 in]
              n235 = case shown="0, Default" w661 {
                tunnel: w660 -> [w668 w671]
                tunnel: w659 -> [_ w670]
                tunnel: [w668 w669] -> w658
                frame 0, Default {
                }
                frame -1 {
                  n236 = Build Array (concatenate)(w671, w670) -> (w669:refnum<vi>[])
                }
              }
            }
            n237 = for {
              tunnel: w649 -> [w657] mode=indexing
              tunnel: [w654] -> w650 mode=indexing
              n238 = property class="LVClassLibrary"(reference=w657) -> ("Name"=w655:string)  [unwired: 1 in, 2 out]
              n239 = Match Pattern(string=w655, regular expression="\\2Elvclass") -> (before substring=w654:string)  [unwired: 1 in, 3 out]
            }
            n240 = Build Array (concatenate)("" ("regular expression"), w650) -> (w648:string[])
            n241 = property on="ParentClass" class="Ring (strict)"("Strings []"=w648) -> ()  [unwired: 2 in, 2 out]
          }
          frame 2 {
            n242 = Unbundle By Name(w691) -> ("Classes"=w689:refnum<vi>[], "Selected"=w690:i32[])
            n243 = Index Array(array=w690) -> (element=w688:i32)  [unwired: 1 in]
            n244 = Delete From Array(array=w689, index=w688) -> (array with subset deleted=w687:refnum<vi>[])  [unwired: 1 in, 1 out]
            n245 = for {
              tunnel: w687 -> [w697] mode=indexing
              tunnel: [w694] -> w693 mode=indexing
              n246 = property class="LVClassLibrary"(reference=w697) -> ("Name"=w695:string)  [unwired: 1 in, 2 out]
              n247 = Match Pattern(string=w695, regular expression="\\2Elvclass") -> (before substring=w694:string)  [unwired: 1 in, 3 out]
            }
            n248 = Build Array (concatenate)("" ("regular expression"), w693) -> (w686:string[])
            n249 = property on="InterfaceClass" class="Ring (strict)"("Strings []"=w686) -> ()  [unwired: 2 in, 2 out]
          }
          frame 1 {
            n250 = Unbundle By Name(w699) -> ("Interfaces"=w698:refnum<vi>[])
            n251 = for {
              tunnel: w698 -> [w706] mode=indexing
              tunnel: [w703] -> w702 mode=indexing
              n252 = property class="LVClassLibrary"(reference=w706) -> ("Name"=w704:string)  [unwired: 1 in, 2 out]
              n253 = Match Pattern(string=w704, regular expression="\\2Elvclass") -> (before substring=w703:string)  [unwired: 1 in, 3 out]
            }
            n254 = Build Array (concatenate)("" ("regular expression"), w702) -> (w701:string[])
            n255 = property on="ParentClass" class="Ring (strict)"("Strings []"=w701) -> ()  [unwired: 2 in, 2 out]
          }
        }
        n256 = Bundle By Name(cluster=w638, "DropDownClasses"=w639) -> (w640:T2)
      }
      frame "UpdateMethods" {
        n257 = Unbundle By Name(w719) -> ("Selected"=w716:i32[], "Classes"=w709:refnum<vi>[], "ExistingParentClassIdx"=w708:i32)
        n258 = Index Array(array=w716) -> (element=w723:i32)  [unwired: 1 in]
        n259 = Empty Array?(array=w716) -> (empty?=w715:bool)
        n260 = Index Array(array=w709, index=w708) -> (element=w707:refnum<vi>)
        n261 = Index Array(array=w709, index=w723) -> (element=w714:refnum<vi>)
        n262 = Select(t=refnum<vi> refnum, s=w715, f=w714) -> (s? t:f=w713:refnum<vi>)
        n263 = feedback-in #1(w713) -> ()
        n264 = feedback #1() -> (w721:refnum<vi>)
        n265 = Not Equal?(x=w714, y=w721) -> (x != y?=w720:bool)
        n266 = Compound Arithmetic op=AND(invert w715, w720) -> (w717:bool)
        n267 = case shown="True" w717 {
          tunnel: w714 -> [_ w735]
          tunnel: w719 -> [w726 w739]
          tunnel: [w726 w737] -> w718
          tunnel: w707 -> [_ w731]
          frame False {
          }
          frame True {
            n268 = invoke class="LVClassLibrary" method="Get All Descendents"(reference=w731, "Type"="VI") -> ("All Descendents"=w730:refnum<vi>[])  [unwired: 5 in, 6 out]
            n269 = invoke class="LVClassLibrary" method="Get All Descendents"(reference=w735, "Type"="VI") -> (reference out=w734:refnum<vi>, "All Descendents"=w740:refnum<vi>[])  [unwired: 5 in, 5 out]
            n270 = for {
              tunnel: w730 -> [w743] mode=indexing
              tunnel: [w742] -> w729 mode=indexing
              n271 = property class="ProjectItem"(reference=w743) -> ("Name"=w742:string)  [unwired: 1 in, 2 out]
            }
            n272 = for {
              tunnel: w740 -> [w762] mode=indexing
              tunnel: [w765] -> w738 mode=indexing if=w744
              tunnel: [w754] -> w733 mode=indexing if=w744
              tunnel: string[] ["_Create\\2Evi$", "^Destroy\\2Evi$", ".ctl$", "_GetObjectStatus.vi", "_GetAttributes.vi", "_New.vi", "_GOOPKernel.vi", "^CleanUp.vi$", "_Init.vi$"] -> [w764]
              tunnel: w734 -> [w763]
              tunnel: w729 -> [w752]
              shift-right: [w749] -> _
              shift-left: 0 -> [w747]
              tunnel: [w747] -> w727 mode=indexing if=w745
              n273 = property class="ProjectItem"(reference=w762) -> (reference out=w765:refnum<vi>, "Name"=w751:string)  [unwired: 1 in, 1 out]
              n274 = invoke class="LVClassLibrary" method="Get Source Scope"(reference=w763, "SourceRef"=w762) -> ("GetSourceScope"=w760:T5)  [unwired: 3 in, 4 out]
              n275 = for {
                tunnel: w751 -> [w769]
                tunnel: [w767] -> w756
                tunnel: w764 -> [w766] mode=indexing
                stop <- w767 stop-if-true
                n276 = Match Pattern(string=w769, regular expression=w766) -> (offset past match=w768:i32)  [unwired: 1 in, 3 out]
                n277 = Greater Or Equal To 0?(x=w768) -> (x >= 0?=w767:bool)
              }
              n278 = Search 1D Array(1D array=w752, element=w751) -> (index of element=w750:i32)  [unwired: 1 in]
              n279 = Equal?(x=T5."public" ("Source Scope:Get"), y=w760) -> (x = y?=w758:bool)
              n280 = Equal?(x=T5."protected" ("Source Scope:Get"), y=w760) -> (x = y?=w757:bool)
              n281 = Match Pattern(string=w751, regular expression="\\2E[victl]+$") -> (before substring=w754:string)  [unwired: 1 in, 3 out]
              n282 = Greater Or Equal To 0?(x=w750) -> (x >= 0?=w746:bool)
              n283 = Or(x=w758, y=w757) -> (x .or. y?=w755:bool)
              n284 = Compound Arithmetic op=AND(w755, invert w756) -> (w744:bool)
              n285 = And(x=w744, y=w746) -> (x .and. y?=w745:bool)
              n286 = Increment(x=w747) -> (x+1=w748:i32)
              n287 = Select(t=w748, s=w744, f=w747) -> (s? t:f=w749:i32)
            }
            n288 = property on="MyClassMethods" class="LstBox (strict)"("Item Names"=w733, "Disabled Items"=w727) -> ()  [unwired: 2 in, 2 out]
            n289 = property on="MyClassMethods(Interface)" class="LstBox (strict)"("Item Names"=w733) -> ()  [unwired: 2 in, 2 out]
            n290 = Bundle By Name(cluster=w739, "Methods"=w738) -> (w737:T2)
          }
        }
        n291 = local read "InterfaceOptionTab"() -> (w711:enum32{"Parent", "Adapter"})
        n292 = case shown="\"Parent\", Default" w711 {
          tunnel: ["ValidateOptions" "UpdateInterfaceMethods"] -> w710
          frame "Parent", Default {
          }
          frame "Adapter" {
          }
        }
      }
      frame "UpdateInterfaceMethods" {
        n293 = local read "MyClassMethods(Interface)"() -> (w771:i32[])
        n294 = property on="MyClassMethods(Interface)" class="LstBox (strict)" props=["Item Names", "Item Symbols"]() -> ("Item Names"=w775:string[])  [unwired: 2 in, 3 out]
        n295 = for {
          tunnel: w775 -> [_] mode=indexing
          tunnel: [w780] -> w774 mode=indexing if=w778
          tunnel: w771 -> [w781]
          i -> [w780]
          n296 = Search 1D Array(1D array=w781, element=w780) -> (index of element=w779:i32)  [unwired: 1 in]
          n297 = Less Than 0?(x=w779) -> (x < 0?=w778:bool)
        }
        n298 = Build Array(w775) -> (w777:string[][])
        n299 = Transpose 2D Array(2D array=w777) -> (transposed array=w776:string[][])
        n300 = property on="Parent Methods" class="MCListbox (strict)"("ItemNames"=w776, "DisabledItems"=w774) -> ()  [unwired: 2 in, 2 out]
      }
      frame "AutoUpdateAdaptorName" {
        n301 = Unbundle By Name(w798) -> ("AdpUpdates"=w797:bool, "SelectClassPath"=w787:path)
        n302 = case shown="False" w797 {
          tunnel: w796 -> [w919 _]
          tunnel: w795 -> [w916 _]
          tunnel: [w915 w934] -> w786
          frame False {
            n303 = local read "InterfaceClassName"() -> (w920:string)
            n304 = Equal?(x=w919, y=w920) -> (x = y?=w918:bool)
            n305 = Empty String/Path?(string/path=w920) -> (empty?=w921:bool)
            n306 = Or(x=w918, y=w921) -> (x .or. y?=w917:bool)
            n307 = case shown="False" w917 {
              tunnel: [w924 w930] -> w922
              tunnel: w920 -> [w925 _]
              tunnel: w916 -> [_ w931]
              tunnel: [w924 _] -> w915
              frame False {
                n308 = property on="AdaptorClassName" class="Str"() -> ("Key Focus"=w923:bool)  [unwired: 2 in, 2 out]
                n309 = case shown="False" w923 {
                  tunnel: w925 -> [w927 _]
                  tunnel: [w926 _] -> w924
                  frame False {
                    n310 = local read "MyClassName(InteraceClass)"() -> (w928:string)
                    n311 = Format Into String(format string="%s_%s", w927, w928) -> (resulting string=w926:string)  [unwired: 2 in, 1 out]
                  }
                  frame True {
                  }
                }
              }
              frame True {
                n312 = property on="AdaptorClassName" class="Str"() -> ("Key Focus"=w932:bool)  [unwired: 2 in, 2 out]
                n313 = case shown="True" w932 {
                  tunnel: w931 -> [w933 _]
                  tunnel: [w933 _] -> w930
                  frame False {
                  }
                  frame True {
                  }
                }
              }
            }
            n314 = local write "AdaptorClassName"(w922) -> ()
          }
          frame True {
            n315 = local read "AdaptorClassName"() -> (w934:string)
          }
        }
        n316 = Strip Path(path=w787) -> (stripped path=w788:path)  [unwired: 1 out]
        n317 = Strip Path(path=w788) -> (stripped path=w794:path, name=w789:string)
        n318 = xnode "Match Regular Expression"("input string"=w789, "regular expression"="_class$", "ignore case? (F)"=TRUE) -> ("whole match"=w793:string)  [unwired: 3 in, 4 out]
        n319 = Concatenate Strings(w786, w793) -> (w792:string)
        n320 = Empty String/Path?(string/path=w786) -> (empty?=w785:bool)
        n321 = Build Path(base path=w794, name or relative path=w792) -> (appended path=w784:path)
        n322 = Select(t=path "", s=w785, f=w784) -> (s? t:f=w783:path)
        n323 = local write "AdaptorFolder"(w783) -> ()
      }
      frame "ValidateOptions" {
        (unwired) enum32{"Parent", "Adapter"}."Parent" ("InterfaceOptionTab")
        n324 = local read "InterfaceOptionTab"() -> (w938:enum32{"Parent", "Adapter"})
        n325 = case shown="\"Adapter\"" w938 {
          tunnel: w937 -> [w945 w997]
          tunnel: w936 -> [w955 w1006]
          tunnel: w935 -> [w954 _]
          frame "Parent", Default {
            w963 = FALSE  # F=Allow No Methods to be selected
            n326 = Unbundle By Name(w945) -> ("ExistingParentClassIdx"=w960:i32)
            n327 = Unbundle By Name(w945) -> ("ExistingParentClassIdx"=w952:i32)
            n328 = property on="ParentFolder" class="Path"() -> ("DisabledEnum"=w950:T4)  [unwired: 2 in, 2 out]
            n329 = Unbundle By Name(w945) -> ("Selected"=w944:i32[])
            n330 = local read "ParentFolder"() -> (w959:path)
            n331 = local read "ParentClassName"() -> (w980:string)
            n332 = local read "InterfaceToCreate"() -> (w970:u16)
            n333 = Equal?(x=w950, y=T4."Enabled" ("Disabled")) -> (x = y?=w948:bool)
            n334 = local read "MyClassMethods"() -> (w964:i32[])
            n335 = Empty Array?(array=w944) -> (empty?=w943:bool)
            n336 = Empty String/Path?(string/path=w980) -> (empty?=w977:bool)
            n337 = Equal?(x=w955, y=w980) -> (x = y?=w979:bool)
            n338 = Equal?(x=w954, y=w980) -> (x = y?=w978:bool)
            n339 = case shown="True" w948 {
              tunnel: [_ w981] -> w947
              frame False {
              }
              frame True {
                n340 = local read "ParentFolder"() -> (w984:path)
                n341 = List Folder(path=w984) -> (filenames=w983:string[])  [unwired: 3 in, 3 out]
                n342 = Array Size(array=w983) -> (size(s)=w982:i32)
                n343 = Greater Than 0?(x=w982) -> (x > 0?=w981:bool)
              }
            }
            n344 = Empty String/Path?(string/path=w959) -> (empty?=w958:bool)
            n345 = Less Than 0?(x=w960) -> (x < 0?=w951:bool)
            n346 = Less Than 0?(x=w952) -> (x < 0?=w953:bool)
            n347 = Compound Arithmetic op=AND(w951, w958) -> (w957:bool)
            n348 = Compound Arithmetic op=OR(w979, w978, w977) -> (w976:bool)
            n349 = Compound Arithmetic op=AND(w951, w953) -> ()  [unwired: 1 out]
            n350 = case shown="0, Default" w970 {
              tunnel: ["The Interface name can't be empty" ("ParentClassName") "The Parent name can't be empty" ("ParentClassName")] -> w969
              frame 1 {
              }
              frame 0, Default {
              }
            }
            n351 = Empty Array?(array=w964) -> ()  [unwired: 1 out]
            n352 = Build Array(w976, w963, w957, w947) -> (w974:bool[])
            n353 = Build Array(w969, "No method(s) have been selected" ("ParentClassName"), "Class folder can't be empty" ("ParentClassName"), "Class folder is not empty" ("ParentClassName")) -> (w962:string[])
            n354 = for {
              tunnel: w974 -> [w987] mode=indexing
              tunnel: w962 -> [w988] mode=indexing
              tunnel: [w988] -> w968 mode=indexing if=w987
            }
            n355 = Array To Spreadsheet String(delimiter (Tab)=", ", array=w968, 3:"%s" ("format string")) -> (spreadsheet string=w965:string)
            n356 = Or Array Elements(Boolean array=w974) -> (logical OR=w973:bool)
            n357 = call <vilib>:"Trim Whitespace.vi"("string"=w965) -> ("trimmed string"=w941:string)  [unwired: 1 in]
            n358 = Select(t="No class selected", s=w943, f=w941) -> (s? t:f=→"ReasonWhyParentClassCan'tBeCreated":string)
            n359 = Select(t=T4."Disabled and Grayed Out" ("Disabled"), s=w973, f=T4."Enabled" ("Disabled")) -> (s? t:f=w975:T4)
            n360 = property on="CreateClassAndMethods" class="Bool"("DisabledEnum"=w975) -> ()  [unwired: 2 in, 2 out]
          }
          frame "Adapter" {
            n361 = Unbundle By Name(w997) -> ("ExistingParentClassIdx"=w1010:i32)
            n362 = Unbundle By Name(w997) -> ("ExistingParentClassIdx"=w1004:i32)
            n363 = property on="InterfaceFolder" class="Path"() -> ("DisabledEnum"=w1002:T4)  [unwired: 2 in, 2 out]
            n364 = Unbundle By Name(w997) -> ("Selected"=w996:i32[])
            n365 = local read "InterfaceFolder"() -> (w989:path)
            n366 = local read "InterfaceClassName"() -> (w991:string)
            n367 = local read "MyClassMethods(Interface)"() -> (w990:i32[])
            n368 = Equal?(x=w1002, y=T4."Enabled" ("Disabled")) -> (x = y?=w1000:bool)
            n369 = Empty Array?(array=w996) -> (empty?=w995:bool)
            n370 = Empty String/Path?(string/path=w991) -> (empty?=w1025:bool)
            n371 = Equal?(x=w1006, y=w991) -> (x = y?=w1026:bool)
            n372 = case shown="True" w1000 {
              tunnel: [_ w1027] -> w999
              frame False {
              }
              frame True {
                n373 = local read "InterfaceFolder"() -> (w1030:path)
                n374 = List Folder(path=w1030) -> (filenames=w1029:string[])  [unwired: 3 in, 3 out]
                n375 = Array Size(array=w1029) -> (size(s)=w1028:i32)
                n376 = Greater Than 0?(x=w1028) -> (x > 0?=w1027:bool)
              }
            }
            n377 = Empty String/Path?(string/path=w989) -> (empty?=w1009:bool)
            n378 = Less Than 0?(x=w1010) -> (x < 0?=w1003:bool)
            n379 = Less Than 0?(x=w1004) -> (x < 0?=w1005:bool)
            n380 = Compound Arithmetic op=AND(w1003, w1009) -> (w1008:bool)
            n381 = Compound Arithmetic op=OR(w1026, w1025) -> (w1024:bool)
            n382 = Compound Arithmetic op=AND(w1003, w1005) -> ()  [unwired: 1 out]
            n383 = Empty Array?(array=w990) -> (empty?=w1013:bool)
            n384 = Build Array(w1024, w1013, w1008, w999) -> (w1022:bool[])
            n385 = Build Array("The Parent name can't be empty" ("ParentClassName"), "No method(s) have been selected" ("ParentClassName"), "Parent class folder can't be empty" ("ParentClassName"), "Parent class folder is not empty" ("ParentClassName")) -> (w1012:string[])
            n386 = for {
              tunnel: w1022 -> [w1031] mode=indexing
              tunnel: w1012 -> [w1032] mode=indexing
              tunnel: [w1032] -> w1017 mode=indexing if=w1031
            }
            n387 = Array To Spreadsheet String(delimiter (Tab)=", ", array=w1017, 3:"%s" ("format string")) -> (spreadsheet string=w1014:string)
            n388 = Or Array Elements(Boolean array=w1022) -> (logical OR=w1021:bool)
            n389 = call <vilib>:"Trim Whitespace.vi"("string"=w1014) -> ("trimmed string"=w994:string)  [unwired: 1 in]
            n390 = Select(t="No class selected", s=w995, f=w994) -> (s? t:f=→"ReasonWhyInterfaceClassCan'tBeCreated":string)
            n391 = Select(t=T4."Disabled and Grayed Out" ("Disabled"), s=w1021, f=T4."Enabled" ("Disabled")) -> (s? t:f=w1023:T4)
            n392 = property on="CreateInterfaceAdaptorClassAndMethods" class="Bool"("DisabledEnum"=w1023) -> ()  [unwired: 2 in, 2 out]
          }
        }
      }
      frame "UpdateCP" {
        w1049 = u32[] []
        # "444=4815\n565=4833\n686=4834"
        n393 = Unbundle By Name(w1052) -> ("Classes"=w1051:refnum<vi>[], "Selected"=w1050:i32[])
        n394 = for {
          tunnel: w1051 -> [w1072]
          tunnel: w1050 -> [w1071] mode=indexing
          shift-right: [w1065] -> w1048
          shift-left: w1049 -> [w1066]
          shift-right: [w1063] -> w1042
          shift-left: w1049 -> [w1064]
          n395 = Index Array(array=w1072, index=w1071) -> (element=w1070:refnum<vi>)
          n396 = property class="LVClassLibrary"(reference=w1070) -> ("Dynamic Member VIs"=w1069:refnum<vi>[], "Static Member VIs"=w1068:refnum<vi>[])  [unwired: 1 in, 2 out]
          n397 = Build Array (concatenate)(w1069, w1068) -> (w1067:refnum<vi>[])
          n398 = for {
            tunnel: w1067 -> [w1082] mode=indexing
            shift-right: [w1075] -> w1065
            shift-left: w1066 -> [w1077]
            shift-right: [w1073] -> w1063
            shift-left: w1064 -> [w1074]
            n399 = property class="VI"(reference=w1082) -> (reference out=w1079:refnum<vi>, "ConPane"=w1081:refnum<vi>)  [unwired: 1 in, 1 out]
            n400 = property class="ConPane"(reference=w1081) -> (error out=w1080:errorcluster, "Pattern"=w1076:u32)  [unwired: 1 in, 1 out]
            n401 = Search 1D Array(1D array=w1077, element=w1076) -> (index of element=w1078:i32)  [unwired: 1 in]
            n402 = case shown="-1" w1078 {
              selector: w1078 -> [w1083 _]
              tunnel: w1077 -> [w1086 w1093]
              tunnel: w1076 -> [_ w1094]
              tunnel: [w1086 w1092] -> w1075
              tunnel: w1074 -> [w1085 w1090]
              tunnel: [w1084 w1089] -> w1073
              frame 0, Default {
                n403 = in-place {
                  n404 = in-place-array #2(w1085, w1083) -> (w1088:u32)
                  n405 = Increment(x=w1088) -> (x+1=w1087:u32)
                  n406 = in-place-array #2(w1087) -> (w1084:u32[])  [unwired: 1 out]
                }
              }
              frame -1 {
                n407 = Build Array (concatenate)(w1093, w1094) -> (w1092:u32[])
                n408 = Build Array (concatenate)(w1090, u32 1 ("Pattern")) -> (w1089:u32[])
              }
            }
            n409 = Close Reference(reference=w1079, error in (no error)=w1080) -> ()  [unwired: 1 out]
          }
        }
        n410 = Array Size(array=w1042) -> (size(s)=w1041:i32)
        n411 = Array Max & Min(array=w1042) -> (max index (indices)=w1047:i32)  [unwired: 3 out]
        n412 = Index Array(array=w1048, index=w1047) -> (element=w1046:u32)
        n413 = Greater?(x=w1041, y=1) -> (0:w1037:bool)
        n414 = case shown="4815, Default" w1046 {
          tunnel: [w1056 w1059 w1062] -> w1043
          tunnel: [0 1 2] -> w1039
          tunnel: [w1054 w1058 w1061] -> w1038
          frame 4815, Default {
            w1054 = u16 2 items=["4x4x4", "5x6x5", "6x8x6"] ("CP2")
            w1056 = T1 0 items=["4x4x4", "5x6x5", "6x8x6"] ("CP1")
          }
          frame 4833 {
            w1058 = u16 2 items=["4x4x4", "5x6x5", "6x8x6"] ("CP2")
            w1059 = T1 1 items=["4x4x4", "5x6x5", "6x8x6"] ("CP1")
          }
          frame 4834 {
            w1061 = u16 0 items=["4x4x4", "5x6x5", "6x8x6"] ("CP2")
            w1062 = T1 2 items=["4x4x4", "5x6x5", "6x8x6"] ("CP1")
          }
        }
        n415 = Select(t=T4."Disabled and Grayed Out", s=w1037, f=T4."Enabled" ("Disabled")) -> (s? t:f=w1033:T4)
        n416 = property on="CP1" class="Ring (strict)"("Value"=w1043, "DisabledEnum"=w1033) -> ()  [unwired: 2 in, 2 out]
        n417 = Build Array(w1039) -> (w1036:i32[])
        n418 = Select(t=i32[] [], s=w1037, f=w1036) -> (s? t:f=w1035:i32[])
        n419 = property on="CP2" class="Ring (strict)"("Disabled Items []"=w1035, "Value"=w1038) -> ()  [unwired: 2 in, 2 out]
      }
      frame "", "Idle" {
        n420 = event shown="[16] \"CreateInterfaceAdaptorClassAndMethods\", \"CreateClassAndMethods\": Value Change" {
          selector: _ -> [_ _ _ _ _ _ _ _ _ _ _ _ _ _ _ _ _ _ _ _ _ _ _]
          dyn-events: _ -> [_ _ _ _ _ _ _ _ _ _ _ _ _ _ _ _ _ _ _ _ _ _ _]
          timeout: 100 -> [_ _ _ _ _ _ _ _ _ _ _ _ _ _ _ _ _ _ _ _ _ _ _]
          tunnel: w1099 -> [w1111 w1121 w1122 w1126 w1130 w1142 w1168 w1178 w1195 w1213 w1221 w1240 w1370 w1387 w1403 w1418 w1421 w1425 w1426 w1432 w1449 w1468 w1475]
          tunnel: [w1109 w1121 w1122 w1126 w1130 w1142 w1166 w1178 w1181 w1201 w1221 w1240 w1366 w1382 w1403 w1418 w1421 w1425 w1426 w1431 w1449 w1468 w1475] -> w1104
          tunnel: ["Update" "ApplyCp" "Exit" "UpdateClassControl" w1128 "Idle" "Update" "ValidateOptions" "ValidateOptions" "AutoUpdateAdaptorName" "UpdateInterfaceTab" "ValidateOptions" "UpdateInterfaceTab" "UpdateInterfaceTab" w1402 "UpdateInterfaceTab" w1419 "UpdateInterfaceMethods" _ _ "UpdateClassControlNames" _ _] -> w1103
          tunnel: w1101 -> [w1113 _ _ _ _ w1145 _ _ _ _ _ _ _ _ _ _ _ _ _ _ _ _ _]
          tunnel: w1100 -> [w1112 _ _ _ _ w1144 _ _ _ _ _ _ _ _ _ _ _ _ _ _ _ _ _]
          tunnel: w1099 -> [w1108 _ _ _ _ _ w1155 _ w1194 w1212 _ _ w1363 _ _ _ _ _ _ _ _ _ _]
          tunnel: w1098 -> [_ _ _ _ _ _ _ _ _ _ w1219 _ w1374 _ _ _ _ _ _ _ _ _ _]
          tunnel: w1096 -> [_ _ _ _ _ _ _ _ _ _ w1216 _ w1372 _ _ _ _ _ _ _ _ _ _]
          tunnel: w1095 -> [_ _ _ _ _ _ _ _ _ _ _ _ _ w1384 _ _ _ _ _ _ _ _ _]
          event "ClassesOK", "ClassesCancel": Value Change {
            n421 = event-data() -> ()  [unwired: 1 in, 1 out]
            n422 = Unbundle By Name(w1108) -> ("Selected"=w1106:i32[])
            n423 = case shown="True" "ClassesOK" {
              tunnel: w1106 -> [w1114 _]
              tunnel: [w1114 w1115] -> w1105
              frame False {
                n424 = local write "Classes"(w1114) -> ()
              }
              frame True {
                n425 = local read "Classes"() -> (w1115:i32[])
              }
            }
            n426 = for {
              tunnel: w1113 -> [w1119] mode=indexing
              n427 = property on="Property Node" class="Ctl"(reference=w1119, "Visible"=FALSE) -> ()  [unwired: 1 in, 2 out]
            }
            n428 = for {
              tunnel: w1112 -> [w1117] mode=indexing
              n429 = property on="Property Node" class="Ctl"(reference=w1117, "Visible"=TRUE) -> ()  [unwired: 1 in, 2 out]
            }
            n430 = Bundle By Name(cluster=w1111, "Selected"=w1105) -> (w1109:T2)
          }
          event "ApplyCP": Value Change {
            n431 = event-data() -> ()  [unwired: 1 in, 6 out]
          }
          event Panel Close? {
            n432 = event-data() -> ()  [unwired: 1 in, 1 out]
            n433 = event-data("Discard?"=TRUE) -> ()  [unwired: 1 in, 1 out]
          }
          event "ClassControlName": Value Change {
            n434 = event-data() -> ()  [unwired: 1 in, 2 out]
          }
          event "Tab": Value Change {
            (unwired) enum32{"CP", "ClassControlName", "Interface"}."ClassControlName" ("Tab")
            n435 = event-data() -> ()  [unwired: 1 in, 2 out]
            n436 = case shown="\"CP\", Default" "Tab" {
              tunnel: ["UpdateCP" "UpdateClassControl" "CheckClassSelection"] -> w1128
              tunnel: [TRUE TRUE _] -> w1127
              frame "CP", Default {
              }
              frame "ClassControlName" {
              }
              frame "Interface" {
              }
            }
            n437 = property on="MoreClasses" class="Bool"("Visible"=w1127) -> ()  [unwired: 2 in, 2 out]
          }
          event "MoreClasses": Value Change {
            n438 = event-data() -> ()  [unwired: 1 in, 2 out]
            n439 = local read "Classes"() -> (w1141:i32[])
            n440 = property on="Classes" class="LstBox (strict)"() -> ("Top Row"=w1138:i32)  [unwired: 2 in, 2 out]
            n441 = Index Array(array=w1141) -> (element=w1136:i32)  [unwired: 1 in]
            n442 = for {
              tunnel: w1145 -> [w1150] mode=indexing
              n443 = property on="Property Node" class="Ctl"(reference=w1150, "Visible"=TRUE) -> ()  [unwired: 1 in, 2 out]
            }
            n444 = for {
              tunnel: w1144 -> [w1148] mode=indexing
              n445 = property on="Property Node" class="Ctl"(reference=w1148, "Visible"=FALSE) -> ()  [unwired: 1 in, 2 out]
            }
            n446 = Add(x=w1138, y=32) -> (x+y=w1139:i32)
            n447 = In Range and Coerce(upper limit=w1139, x=w1136, lower limit=w1138) -> (In Range?=w1137:bool)  [unwired: 1 out]
            n448 = case shown="False" w1137 {
              tunnel: w1136 -> [w1146 _]
              frame False {
                n449 = property on="Classes" class="LstBox (strict)"("Top Row"=w1146) -> ()  [unwired: 2 in, 2 out]
              }
              frame True {
              }
            }
          }
          event "Class(es)": Value Change {
            w1156 = T4."Enabled" ("Disabled")
            w1158 = path "" ("ParentFolder")
            w1159 = 0 ("Classes")
            w1157 = "" ("Caption.Text")
            n450 = event-data() -> ()  [unwired: 1 in, 2 out]
            n451 = Unbundle By Name(w1155) -> ("Classes"=w1154:refnum<vi>[])
            n452 = Subtract(x="Class(es)", y=u16 2) -> (x-y=w1153:u16)
            n453 = local write "ParentClassName"(w1157) -> ()
            n454 = case shown="0.." w1153 {
              selector: w1153 -> [_ w1171]
              frame Default {
              }
              frame 0.. {
                n455 = property on="Classes" class="LstBox (strict)"() -> ("Item Names"=w1174:string[])  [unwired: 2 in, 2 out]
                n456 = Index Array(array=w1174, index=w1171) -> (element=w1175:string)
                n457 = Build Array (concatenate)(w1175, "-" ("element"), w1174) -> (w1173:string[])
                n458 = property on="Class(es)" class="Ring (strict)"("Strings []"=w1173, "Value"=0 ("Classes")) -> ()  [unwired: 2 in, 2 out]
              }
            }
            n459 = local write "ParentFolder"(w1158) -> ()
            n460 = local write "ParentClass"(w1159) -> ()
            n461 = Index Array(array=w1154, index=w1153) -> (element=w1152:refnum<vi>)
            n462 = property class="LVClassLibrary"(reference=w1152) -> ("Path"=w1151:path)  [unwired: 1 in, 2 out]
            n463 = local write "InterfaceClass"(w1159) -> ()
            n464 = local write "InterfaceClassName"(w1157) -> ()
            n465 = local write "InterfaceFolder"(w1158) -> ()
            n466 = Build Array(w1153) -> (w1165:u16[])
            n467 = property on="Classes" class="LstBox (strict)"("Value"=w1165) -> ()  [unwired: 2 in, 2 out]
            n468 = Bundle By Name(cluster=w1168, "SelectClassPath"=w1151, "Selected"=w1165) -> (w1166:T2)
            n469 = property on="InterfaceFolder" class="Path"("DisabledEnum"=w1156) -> ()  [unwired: 2 in, 2 out]
            n470 = property on="ParentFolder" class="Path"("DisabledEnum"=w1156) -> ()  [unwired: 2 in, 2 out]
            n471 = property on="Class(es)" class="Ring (strict)"("Caption.Text"="") -> ()  [unwired: 2 in, 2 out]
            n472 = property on="MyClassMethods" class="LstBox (strict)"("Item Names"=string[] [], "Value"=i32[] [] ("MyClassMethods")) -> ()  [unwired: 2 in, 2 out]
            n473 = property on="MyClassMethods(Interface)" class="LstBox (strict)"("Item Names"=string[] [], "Value"=i32[] [] ("MyClassMethods")) -> ()  [unwired: 2 in, 2 out]
          }
          event "MyClassMethods": Value Change {
            n474 = event-data() -> ()  [unwired: 1 in, 2 out]
          }
          event "ParentClass": Value Change {
            n475 = event-data() -> ()  [unwired: 1 in, 2 out]
            n476 = property on="ParentClass" class="Ring (strict)"() -> ("Strings []"=w1192:string[])  [unwired: 2 in, 2 out]
            n477 = Unbundle By Name(w1194) -> ("DropDownClasses"=w1193:refnum<vi>[])
            n478 = Index Array(array=w1192, index="ParentClass") -> (element=w1189:string)
            n479 = Decrement(x="ParentClass") -> (x-1=w1180:u16)
            n480 = Index Array(array=w1193, index=w1180) -> (element=w1188:refnum<vi>)
            n481 = property class="LVClassLibrary"(reference=w1188) -> ("Path"=w1182:path)  [unwired: 1 in, 2 out]
            n482 = Strip Path(path=w1182) -> (stripped path=w1187:path)  [unwired: 1 out]
            n483 = Empty String/Path?(string/path=w1182) -> (empty?=w1186:bool)
            n484 = Bundle By Name(cluster=w1195, "NewDropDownClassIdx"=w1180) -> (w1181:T2)
            n485 = Select(t=T4."Enabled" ("Disabled"), s=w1186, f=T4."Disabled and Grayed Out" ("Disabled")) -> (s? t:f=w1183:T4)
            n486 = property on="ParentFolder" class="Path"("Value"=w1187, "DisabledEnum"=w1183) -> ()  [unwired: 2 in, 2 out]
            n487 = property on="ParentClassName" class="Str"("Text.TextColor"=u32 0, "Value"=w1189, "DisabledEnum"=w1183) -> ()  [unwired: 2 in, 2 out]
          }
          event "InterfaceClass": Value Change {
            n488 = event-data() -> ()  [unwired: 1 in, 2 out]
            n489 = property on="InterfaceClass" class="Ring (strict)"() -> ("Strings []"=w1210:string[])  [unwired: 2 in, 2 out]
            n490 = Unbundle By Name(w1212) -> ("DropDownClasses"=w1211:refnum<vi>[])
            n491 = Index Array(array=w1210, index="InterfaceClass") -> (element=w1197:string)
            n492 = Decrement(x="InterfaceClass") -> (x-1=w1200:u16)
            n493 = Index Array(array=w1211, index=w1200) -> (element=w1208:refnum<vi>)
            n494 = property class="LVClassLibrary"(reference=w1208) -> ("Path"=w1202:path)  [unwired: 1 in, 2 out]
            n495 = Strip Path(path=w1202) -> (stripped path=w1207:path)  [unwired: 1 out]
            n496 = Empty String/Path?(string/path=w1202) -> (empty?=w1206:bool)
            n497 = Bundle By Name(cluster=w1213, "AdpUpdates"=FALSE, "NewDropDownClassIdx"=w1200) -> (w1201:T2)
            n498 = Select(t=T4."Enabled" ("Disabled"), s=w1206, f=T4."Disabled and Grayed Out" ("Disabled")) -> (s? t:f=w1203:T4)
            n499 = property on="InterfaceFolder" class="Path"("Value"=w1207, "DisabledEnum"=w1203) -> ()  [unwired: 2 in, 2 out]
            n500 = property on="InterfaceClassName" class="Str"("Text.TextColor"=u32 0, "Value"=w1197, "DisabledEnum"=w1203) -> ()  [unwired: 2 in, 2 out]
          }
          event "ParentClassName": Value Change; "ParentClassName": Mouse Down {
            n501 = event-data() -> ("Type"=w1220:T20)  [unwired: 1 in, 1 out]
            n502 = case shown="\"Mouse Down\"" w1220 {
              tunnel: w1219 -> [_ w1228]
              tunnel: "ParentClassName" -> [_ w1225]
              tunnel: w1216 -> [_ w1226]
              frame "Null", Default {
              }
              frame "Mouse Down" {
                n503 = Equal?(x=w1228, y=w1225) -> (x = y?=w1222:bool)
                n504 = Equal?(x=w1226, y=w1225) -> (x = y?=w1223:bool)
                n505 = Or(x=w1222, y=w1223) -> (x .or. y?=w1224:bool)
                n506 = property on="ParentClassName" class="Str"("Key Focus"=TRUE) -> ()  [unwired: 2 in, 2 out]
                n507 = case shown="False" w1224 {
                  frame False {
                  }
                  frame True {
                    n508 = local write "ParentClassName"("" ("ParentClassName")) -> ()
                  }
                }
              }
            }
            n509 = property on="ParentClassName" class="Str"("Text.TextColor"=u32 0) -> ()  [unwired: 2 in, 2 out]
            n510 = property on="ParentClassName" class="Str"("Text.TextColor"=u32 0) -> ()  [unwired: 2 in, 2 out]
          }
          event "ParentFolder": Value Change {
            n511 = event-data() -> ()  [unwired: 1 in, 6 out]
            n512 = Strip Path(path="ParentFolder") -> (name=w1239:string)  [unwired: 1 out]
            n513 = local read "ParentClassName"() -> (w1232:string)
            n514 = xnode "Match Regular Expression"("input string"=w1239, "regular expression"="_class$", "ignore case? (F)"=TRUE) -> ("before match"=w1236:string)  [unwired: 3 in, 4 out]
            n515 = To Lower Case(string=w1232) -> (all lower case string=w1235:string)
            n516 = To Lower Case(string=w1236) -> (all lower case string=w1234:string)
            n517 = Equal?(x=w1235, y=w1234) -> (x = y?=w1233:bool)
            n518 = case shown="False" w1233 {
              tunnel: w1232 -> [w1246 _]
              tunnel: "ParentFolder" -> [w1242 _]
              frame False {
                n519 = Empty String/Path?(string/path=w1242) -> (empty?=w1241:bool)
                n520 = Concatenate Strings(w1246, "_class" ("regular expression")) -> (w1244:string)
                n521 = Build Path(base path=w1242, name or relative path=w1244) -> (appended path=w1243:path)
                n522 = case shown="False" w1241 {
                  tunnel: w1243 -> [w1247 _]
                  frame False {
                    n523 = local write "ParentFolder"(w1247) -> ()
                  }
                  frame True {
                  }
                }
              }
              frame True {
              }
            }
          }
          event "InterfaceClassName": Mouse Down; "InterfaceClassName": Value Change {
            n524 = event-data() -> ("Type"=w1365:T20)  [unwired: 1 in, 1 out]
            n525 = Unbundle By Name(w1363) -> ("AdpUpdates"=w1362:bool)
            n526 = Equal?(x=w1374, y="InterfaceClassName") -> (x = y?=w1367:bool)
            n527 = Equal?(x=w1372, y="InterfaceClassName") -> (x = y?=w1368:bool)
            n528 = Or(x=w1367, y=w1368) -> (x .or. y?=w1369:bool)
            n529 = case shown="\"Mouse Down\"" w1365 {
              tunnel: w1370 -> [w1375 w1379]
              tunnel: w1369 -> [w1376 _]
              tunnel: [w1375 w1379] -> w1366
              tunnel: "InterfaceClassName" -> [_ _]
              tunnel: w1362 -> [_ _]
              frame "Mouse Down" {
                n530 = case shown="True" w1376 {
                  frame False {
                  }
                  frame True {
                    n531 = local write "InterfaceClassName"("" ("ParentClassName")) -> ()
                  }
                }
                n532 = property on="InterfaceClassName" class="Str"("Key Focus"=TRUE) -> ()  [unwired: 2 in, 2 out]
              }
              frame "Value Change", Default {
              }
            }
            n533 = property on="InterfaceClassName" class="Str"("Text.TextColor"=u32 0) -> ()  [unwired: 2 in, 2 out]
          }
          event "AdaptorClassName": Value Change; "AdaptorClassName": Mouse Down {
            n534 = event-data() -> ("Type"=w1381:T20)  [unwired: 1 in, 1 out]
            n535 = Equal?(x=w1384, y="AdaptorClassName") -> (x = y?=w1383:bool)
            n536 = case shown="\"Mouse Down\"" w1381 {
              tunnel: w1387 -> [w1388 w1399]
              tunnel: w1383 -> [w1389 w1393]
              tunnel: [w1388 w1398] -> w1382
              tunnel: "AdaptorClassName" -> [_ w1394]
              frame "Mouse Down" {
                n537 = case shown="False" w1389 {
                  frame False {
                  }
                  frame True {
                    n538 = local write "AdaptorClassName"("" ("ParentClassName")) -> ()
                  }
                }
                n539 = property on="AdaptorClassName" class="Str"("Key Focus"=TRUE) -> ()  [unwired: 2 in, 2 out]
              }
              frame "Value Change", Default {
                n540 = call <vilib>:"Trim Whitespace.vi"("string"=w1394) -> ("trimmed string"=w1397:string)  [unwired: 1 in]
                n541 = Empty String/Path?(string/path=w1397) -> (empty?=w1396:bool)
                n542 = Or(x=w1396, y=w1393) -> (x .or. y?=w1395:bool)
                n543 = Not(x=w1395) -> (.not. x?=w1392:bool)
                n544 = Bundle By Name(cluster=w1399, "AdpUpdates"=w1392) -> (w1398:T2)
              }
            }
            n545 = property on="AdaptorClassName" class="Str"("Text.TextColor"=u32 0) -> ()  [unwired: 2 in, 2 out]
          }
          event Timeout {
            n546 = event-data() -> ()  [unwired: 1 in, 3 out]
            n547 = local read "InterfaceOptionTab"() -> (w1400:enum32{"Parent", "Adapter"})
            n548 = case shown="\"Parent\", Default" w1400 {
              tunnel: [w1404 w1410] -> w1401
              frame "Parent", Default {
                n549 = local read "ParentClassName"() -> (w1406:string)
                n550 = Empty String/Path?(string/path=w1406) -> (empty?=w1405:bool)
                n551 = Compound Arithmetic op=AND(w1405) -> (w1404:bool)
              }
              frame "Adapter" {
                n552 = property on="ParentMethodName" class="Str"() -> ("Key Focus"=w1407:bool)  [unwired: 2 in, 2 out]
                n553 = local read "InterfaceClassName"() -> (w1412:string)
                n554 = local read "AdaptorClassName"() -> (w1409:string)
                n555 = case shown="False" w1407 {
                  frame False {
                    n556 = property on="ParentMethodName" class="Str"("Visible"=FALSE) -> ()  [unwired: 2 in, 2 out]
                  }
                  frame True {
                  }
                }
                n557 = Empty String/Path?(string/path=w1412) -> (empty?=w1411:bool)
                n558 = Empty String/Path?(string/path=w1409) -> (empty?=w1408:bool)
                n559 = Compound Arithmetic op=OR(w1411, w1408) -> (w1410:bool)
              }
            }
            n560 = case shown="False" w1401 {
              tunnel: [_ "UpdateInterfaceTab"] -> w1402
              frame False {
              }
              frame True {
              }
            }
          }
          event "InterfaceToCreate": Value Change {
            n561 = event-data() -> ()  [unwired: 1 in, 6 out]
            n562 = local write "ParentClassName"("" ("ParentClassName")) -> ()
            n563 = local write "ParentFolder"(path "" ("ParentFolder")) -> ()
          }
          event "CreateInterfaceAdaptorClassAndMethods", "CreateClassAndMethods": Value Change {
            n564 = event-data() -> ()  [unwired: 1 in, 1 out]
            n565 = case shown="False" "CreateInterfaceAdaptorClassAndMethods" {
              tunnel: ["CreateParentClass" _] -> w1419
              frame False {
                n566 = call <vilib>:"Set Busy.vi"() -> ()  [unwired: 10 in, 2 out]
              }
              frame True {
                n567 = One Button Dialog(message="Sorry\nThis feature has not been implemented yet.\nBut let me know if this feature would be valuable for you.\nmikael@holmstroms.eu") -> ()  [unwired: 1 in, 1 out]
              }
            }
          }
          event "MyClassMethods(Interface)": Value Change {
            n568 = event-data() -> ()  [unwired: 1 in, 6 out]
          }
          event "SelectAll": Value Change {
            n569 = event-data() -> ()  [unwired: 1 in, 2 out]
            n570 = property on="Classes" class="LstBox (strict)"() -> ("Item Names"=w1429:string[])  [unwired: 2 in, 2 out]
            n571 = Array Size(array=w1429) -> (size(s)=w1428:i32)
            n572 = for {
              N: w1428 -> [_]
              tunnel: [w1430] -> w1427 mode=indexing
              i -> [w1430]
            }
            n573 = property on="Classes" class="LstBox (strict)"("Value"=w1427) -> ()  [unwired: 2 in, 2 out]
          }
          event Key Down {
            n574 = event-data() -> ("Char"=w1435:i16, "PlatMods.Ctrl"=w1436:bool)  [unwired: 1 in]
            n575 = property on="Classes" class="LstBox (strict)"() -> ("Visible"=w1433:bool)  [unwired: 2 in, 2 out]
            n576 = And(x=w1436, y=w1433) -> (x .and. y?=w1434:bool)
            n577 = case shown="True" w1434 {
              tunnel: w1435 -> [_ w1440]
              tunnel: w1432 -> [w1437 w1439]
              tunnel: [w1437 w1438] -> w1431
              frame False {
              }
              frame True {
                n578 = case shown="65, 97" w1440 {
                  tunnel: w1439 -> [w1441 w1444]
                  tunnel: [w1441 w1443] -> w1438
                  frame 0, Default {
                  }
                  frame 65, 97 {
                    n579 = property on="Classes" class="LstBox (strict)"() -> ("Item Names"=w1446:string[])  [unwired: 2 in, 2 out]
                    n580 = Array Size(array=w1446) -> (size(s)=w1445:i32)
                    n581 = for {
                      N: w1445 -> [_]
                      tunnel: [w1447] -> w1442 mode=indexing
                      i -> [w1447]
                    }
                    n582 = property on="Classes" class="LstBox (strict)"("Value"=w1442) -> ()  [unwired: 2 in, 2 out]
                    n583 = Bundle By Name(cluster=w1444, "Selected"=w1442) -> (w1443:T2)
                  }
                }
              }
            }
          }
          event "UpdateClassControlNames": Value Change {
            n584 = event-data() -> ()  [unwired: 1 in, 6 out]
          }
          event "Parent Methods": Value Change {
            w1452 = TRUE ("Visible")
            n585 = event-data() -> ()  [unwired: 1 in, 1 out]
            n586 = property on="Parent Methods" class="MCListbox (strict)"() -> ("ItemNames"=w1467:string[][], "Position"=w1464:T6, "TopLeft"=w1460:T21)  [unwired: 2 in, 2 out]
            n587 = Unbundle By Name(w1460) -> ("Row"=w1458:u32)
            n588 = Add(x=w1464, y=T6 {"Left"=0, "Top"=18} ("x")) -> (x+y=w1462:T6)
            n589 = Subtract(x="Parent Methods", y=w1458) -> (x-y=w1457:u32)
            n590 = Multiply(x=w1457, y=18 ("Top")) -> (x*y=w1454:u32)
            n591 = Index Array(array=w1467, index (row)="Parent Methods", index (col)=0 ("disabled index (col)")) -> (element=w1465:string)
            n592 = Unbundle By Name(w1462) -> ("Left"=w1463:i32, "Top"=w1455:i32)
            n593 = Add(x=w1455, y=w1454) -> (x+y=w1453:u32)
            n594 = property on="ParentMethodName" class="Str"("Left"=w1463, "Top"=w1453, "Value"=w1465, "Visible"=w1452, "Key Focus"=w1452, "Text.Selection Start"=u32 0 ("Text.Selection:Start"), "Text.Selection End"=u32 999 ("Text.Selection:End")) -> ()  [unwired: 2 in, 2 out]
          }
          event "ParentMethodName": Value Change {
            n595 = event-data() -> ()  [unwired: 1 in, 6 out]
            n596 = local read "Parent Methods"() -> (w1472:i32)
            n597 = property on="Parent Methods" class="MCListbox (strict)"() -> ("ItemNames"=w1470:string[][])  [unwired: 2 in, 2 out]
            n598 = Replace Array Subset(array=w1470, new element="ParentMethodName", index (row)=w1472, index (col)=0 ("disabled index (col)")) -> (w1471:string[][])
            n599 = property on="Parent Methods" class="MCListbox (strict)"("ItemNames"=w1471) -> ()  [unwired: 2 in, 2 out]
            n600 = property on="ParentMethodName" class="Str"("Visible"=FALSE) -> ()  [unwired: 2 in, 2 out]
          }
        }
      }
      frame "CheckClassSelection" {
        n601 = Unbundle By Name(w1480) -> ("Selected"=w1482:i32[])
        n602 = Index Array(array=w1482) -> (element=w1481:i32)  [unwired: 1 in]
        n603 = Build Array(w1481) -> (w1479:i32[])
        n604 = Bundle By Name(cluster=w1480, "Selected"=w1479) -> (w1478:T2)
      }
      frame "UpdateClassControlNames" {
        n605 = Unbundle By Name(w1487) -> ("Classes"=w1489:refnum<vi>[], "Selected"=w1488:i32[])
        n606 = local read "ClassControlName"() -> (w1484:string)
        n607 = for {
          tunnel: w1489 -> [w1495]
          tunnel: w1488 -> [w1491] mode=indexing
          shift-right: [w1493] -> w1483
          shift-left: w1486 -> [w1492]
          tunnel: w1484 -> [w1490]
          n608 = Index Array(array=w1495, index=w1491) -> (element=w1494:refnum<vi>)
          n609 = disable-structure shown="Enabled" {
            disable-tunnel: w1494 -> [w1499 _]
            disable-tunnel: [w1498 _] -> w1493
            disable-tunnel: w1492 -> [w1497 _]
            disable-tunnel: w1490 -> [w1496 _]
            frame Enabled {
              n610 = call "Scripting_RenameClassControlsOfClass.vi"("error in (no error)"=w1497, "ClassControlName"=w1496, "LVClassLibrary in"=w1499) -> ("error out"=w1498:errorcluster)  [unwired: 8 in]
            }
            frame Disabled {
            }
          }
        }
      }
      frame "ApplyCp" {
        n611 = call <vilib>:"Set Busy.vi"("error in (no error)"=w1504) -> ("error out"=w1502:errorcluster)  [unwired: 9 in, 1 out]
        n612 = case shown="2, Default" "CP2" {
          tunnel: [w1526 w1527 w1528] -> w1501
          frame 0 {
            w1526 = T1 0 items=["4x4x4", "5x6x5", "6x8x6"] ("Pattern")
          }
          frame 1 {
            w1527 = T1 1 items=["4x4x4", "5x6x5", "6x8x6"] ("Pattern")
          }
          frame 2, Default {
            w1528 = T1 2 items=["4x4x4", "5x6x5", "6x8x6"] ("Pattern")
          }
        }
        n613 = Unbundle By Name(w1507) -> ("Classes"=w1506:refnum<vi>[], "Selected"=w1505:i32[])
        n614 = for {
          shift-right: [w1515] -> w1503
          shift-left: w1502 -> [w1525]
          tunnel: w1506 -> [w1524]
          tunnel: w1505 -> [w1523] mode=indexing
          tunnel: w1501 -> [w1511]
          n615 = Index Array(array=w1524, index=w1523) -> (element=w1522:refnum<vi>)
          n616 = call "GDSLvClass_ReadClassType.vi"("Class Refnum In"=w1522, "error in (no error)"=w1525) -> ("Class Refnum Out"=w1518:refnum<vi>, "ClassSettings"=w1513:T15, "error out"=w1519:errorcluster)  [unwired: 15 in]
          n617 = Unbundle By Name(w1513) -> ("ClassTemplateUsed"=w1512:string)
          n618 = call "GOOP_TemplateRename.vi"("Pattern"=w1511, "TemplateIn"=w1512) -> ("TemplateOut"=w1510:string)  [unwired: 9 in]
          n619 = Format Into String(w1511) -> (resulting string=w1514:string)  [unwired: 3 in, 1 out]
          n620 = Bundle By Name(cluster=w1513, "ConnectorPanePattern"=w1514, "ClassTemplateUsed"=w1510) -> (w1521:T15)
          n621 = call "GDSLvClass_StoreClassType.vi"("Class Refnum In"=w1518, "ClassSettings"=w1521, "CheckAndFixConnectorPaneType(False)"=TRUE, "error in (no error)"=w1519) -> ("Class Refnum Out"=w1517:refnum<vi>, "error out"=w1516:errorcluster)  [unwired: 14 in]
          n622 = invoke class="LVClassLibrary" method="Save"(reference=w1517, error in=w1516) -> (error out=w1515:errorcluster)  [unwired: 2 in, 3 out]
        }
        n623 = call <vilib>:"Unset Busy.vi"("error in (no error)"=w1503) -> ("error out"=w1500:errorcluster)  [unwired: 10 in]
      }
      frame "UpdateClassControl" {
        n624 = local read "ClassControlName"() -> (w1541:string)
        n625 = Unbundle By Name(w1545) -> ("Selected"=w1543:i32[])
        n626 = Index Array(array=w1543) -> (element=w1542:i32)  [unwired: 1 in]
        n627 = property on="Classes" class="LstBox (strict)"() -> ("Item Names"=w1544:string[])  [unwired: 2 in, 2 out]
        n628 = Index Array(array=w1544, index=w1542) -> (element=w1539:string)
        n629 = Search and Replace String(case sensitive?=TRUE ("ignore case? (F)"), input string=w1541, search string="<ClassName>" ("substring (\"\")"), replace string=w1539) -> (result string=w1537:string)  [unwired: 4 in, 3 out]
        n630 = xnode "Match Regular Expression"("input string"=w1537, "regular expression"="(\\w+)/(\\w+)") -> ("before match"=w1534:string, "after match"=w1532:string, "offset past match"=w1535:i32, "submatch 1"=w1533:string, "submatch 2"=w1531:string)  [unwired: 4 in, 2 out]
        n631 = case shown="0, Default" w1535 {
          tunnel: w1534 -> [w1551 w1553]
          tunnel: w1533 -> [w1552 _]
          tunnel: w1532 -> [w1549 _]
          tunnel: w1531 -> [w1550 _]
          tunnel: [w1548 w1553] -> w1530
          tunnel: [w1547 w1553] -> w1529
          frame 0, Default {
            n632 = Concatenate Strings(w1551, w1552, w1549) -> (w1548:string)
            n633 = Concatenate Strings(w1551, w1550, w1549) -> (w1547:string)
          }
          frame -1 {
          }
        }
        "ClassNameIn" <- w1530
        "ClassNameOut" <- w1529
      }
      frame "--------------------------" {
      }
      frame "CreateParentClass" {
        (unwired) T4."Disabled and Grayed Out" ("Disabled")
        # "Get Class info from selected class"
        # "1) Create Base Class of Same Type as Selected Class\n2) Add/Clone Methods from Selected to Parent\n3) Change seleted class to inherit from Parent"
        n634 = Unbundle By Name(w1690) -> ("Classes"=w1689:refnum<vi>[], "Selected"=w1687:i32[])
        n635 = Index Array(array=w1687) -> (element=w1688:i32)  [unwired: 1 in]
        n636 = Index Array(array=w1689, index=w1688) -> (element=w1677:refnum<vi>)
        n637 = call "GDSLvClass_ReadClassType.vi"("Class Refnum In"=w1677) -> ("ClassSettings"=w1679:T15)  [unwired: 16 in, 2 out]
        n638 = Unbundle By Name(w1679) -> ()  [unwired: 1 out]
        n639 = property class="LVClassLibrary"(reference=w1677) -> ("Parent"=w1680:refnum<vi>)  [unwired: 1 in, 2 out]
        n640 = local read "ParentClassName"() -> (w1673:string)
        n641 = local read "ParentFolder"() -> (w1674:path)
        n642 = Bundle By Name(cluster=T7 {"NewInterfaceFolder"=path "", "InterfaceName"="", "InterfaceDescription"="", "ParentInterfacesFilePath"=[], "FolderSuffix"="", "MethodsToCreate"=[]} ("CreateInterfaceType"), "NewInterfaceFolder"=w1674, "InterfaceName"=w1673) -> (w1691:T7)
        n643 = property on="ParentFolder" class="Path"() -> ("DisabledEnum"=w1681:T4)  [unwired: 2 in, 2 out]
        n644 = case shown="\"Enabled\", Default" w1681 {
          tunnel: w1691 -> [w1692 _]
          tunnel: w1678 -> [w1698 w1704]
          tunnel: w1680 -> [w1697 _]
          tunnel: [w1696 w1704] -> w1686
          tunnel: [w1694 w1699] -> w1683
          tunnel: [TRUE ("KeepLvClassRefOpen(False)") _] -> w1676
          frame "Enabled", Default {
            n645 = call "GDSAPI_CreateInterface.vi"("KeepLvClassRefOpen(False)"=TRUE, "error in (no error)"=w1698, "CreateInterfaceType"=w1692, "ProjectItemToCreateClassUnder"=w1697) -> ("error out"=w1696:errorcluster, "LvClassFileOut"=w1694:path)  [unwired: 5 in, 1 out]
          }
          frame "Disabled and Grayed Out" {
            n646 = local read "ParentFolder"() -> (w1701:path)
            n647 = List Folder(path=w1701, pattern="*.lvclass") -> (filenames=w1702:string[])  [unwired: 2 in, 3 out]
            n648 = Index Array(array=w1702) -> (element=w1700:string)  [unwired: 1 in]
            n649 = Build Path(base path=w1701, name or relative path=w1700) -> (appended path=w1699:path)
          }
        }
        n650 = Close Reference(reference=w1680, error in (no error)=w1686) -> (error out=w1685:errorcluster)
        n651 = Bundle By Name(cluster=w1690, "NewClassCreated"=w1676, "ParentClassCreated"=w1683) -> (w1684:T2)
      }
      frame "CreateParentClass_AddMethods" {
        n652 = local read "MyClassMethods"() -> (w1710:i32[])
        n653 = Unbundle By Name(w1708) -> ("Methods"=w1711:refnum<vi>[])
        n654 = Unbundle By Name(w1708) -> ("ParentClassCreated"=w1707:path)
        n655 = for {
          shift-right: [w1722] -> w1706
          shift-left: w1712 -> [w1723]
          tunnel: w1711 -> [w1720]
          tunnel: w1710 -> [w1719] mode=indexing
          tunnel: w1707 -> [w1717]
          n656 = Index Array(array=w1720, index=w1719) -> (element=w1718:refnum<vi>)
          n657 = property class="ProjectItem"(reference=w1718) -> ("Path"=w1716:path)  [unwired: 1 in, 2 out]
          n658 = call <vilib>:"Get File Extension.vi"("file"=w1716) -> ("filename without extension"=w1715:string)  [unwired: 6 in, 4 out]
          n659 = Path To String(path=w1716) -> (string=w1724:string)
          n660 = Bundle By Name(cluster=T14 {"MethodName"="Method1", "RelativeMethodPath"=path "", "MethodDescription"="", "Scope/Visibility"=enum."Public", "MethodType"=enum."Read Attribute", "RelativeProjectClassPath"="", "DynamicDispatchVi"=TRUE, "OverrideMethod(Path)/PropertyMethod(AttributeName)"=""} ("CreateMethodData"), "OverrideMethod(Path)/PropertyMethod(AttributeName)"=w1724, "MethodName"=w1715) -> (w1725:T14)
          n661 = Build Array(w1725) -> (w1726:T22)
          n662 = call "GDSAPI_CreateMethods.vi"("error in (no error)"=w1723, "Methods"=w1726, "ClassPath(*.lvclass)"=w1717) -> ("error out"=w1722:errorcluster)  [unwired: 6 in, 2 out]
        }
        n663 = local read "InterfaceToCreate"() -> (w1705:u16)
        n664 = case shown="1, Default" w1705 {
          tunnel: ["Done" ("message") "CreateParentClass_ChangeInheritance"] -> w1709
          frame 1, Default {
          }
          frame 0 {
          }
        }
      }
      frame "CreateParentClass_ChangeInheritance" {
        # "Change selected class so it inherits from ny base class"
        n665 = Unbundle By Name(w1731) -> ("NewClassCreated"=w1729:bool, "ExistingParentClassIdx"=w1730:i32)
        n666 = Unbundle By Name(w1731) -> ("ParentClassCreated"=w1739:path)
        n667 = Unbundle By Name(w1731) -> ("Classes"=w1735:refnum<vi>[], "Selected"=w1737:i32[])
        n668 = property on="ParentFolder" class="Path" props=["DisabledEnum"]() -> ()  [unwired: 2 in, 3 out]
        n669 = Index Array(array=w1737) -> (element=w1736:i32)  [unwired: 1 in]
        n670 = Index Array(array=w1735, index=w1736) -> (element=w1738:refnum<vi>)
        n671 = Greater Or Equal To 0?(x=w1730) -> (x >= 0?=w1728:bool)
        n672 = Or(x=w1729, y=w1728) -> (x .or. y?=w1727:bool)
        n673 = property class="LVClassLibrary"(reference=w1738) -> ("Path"=w1734:path)  [unwired: 1 in, 2 out]
        n674 = case shown="True" w1727 {
          tunnel: w1740 -> [w1744 w1745]
          tunnel: [w1743 w1745] -> w1733
          tunnel: w1739 -> [w1742 _]
          tunnel: w1734 -> [w1741 _]
          frame True {
            n675 = call "GDSAPI_ChangeInheritance.vi"("error in (no error)"=w1744, "NewParentClassPath(*.lvclass), leave empty to make it a base class"=w1742, "ClassPath(*.lvclass)"=w1741) -> ("error out"=w1743:errorcluster)  [unwired: 7 in, 1 out]
          }
          frame False {
          }
        }
      }
      frame "Done" {
        n676 = call <vilib>:"Unset Busy.vi"() -> ("error out"=w1746:errorcluster)  [unwired: 11 in]
        n677 = flat-sequence {
          tunnel: w1746 -> [_]
          frame #0 {
            n678 = One Button Dialog(message="Done") -> ()  [unwired: 1 in, 1 out]
          }
        }
      }
    }
    n679 = Select(t="Error", s=w46, f=w47) -> (s? t:f=w49:string)
  }
  "Error Out" <- w28
  n680 = Unbundle By Name(w1) -> ("Classes"=w16:refnum<vi>[], "Methods"=w4:refnum<vi>[], "DropDownClasses"=w3:refnum<vi>[], "Interfaces"=w2:refnum<vi>[])
  n681 = Close Reference(reference=w16) -> ()  [unwired: 1 in, 1 out]
  n682 = Close Reference(reference=w4) -> ()  [unwired: 1 in, 1 out]
  n683 = Close Reference(reference=w3) -> ()  [unwired: 1 in, 1 out]
  n684 = Close Reference(reference=w2) -> ()  [unwired: 1 in, 1 out]
